vi "DialogRenameVI.vi"(0 "ObjectIn":refnum<class "ClassWriterNative.lvclass">, 1 "ProjectItem":refnum<vi>, 5 "error in (no error)":errorcluster) -> (14 "ObjectOut":refnum<class "ClassWriterNative.lvclass">, 15 "Cancelled":bool, 16 "RenameOption":T1, 19 "error out":errorcluster)   [LabVIEW 2020, in "ClassWriterNative.lvclass"]
uses:
  <resource>/Framework/Providers/Open_GDS/ClassProviders/Provider_LvNativeClass/ClassWriterNative_class/ClassWriterNative.lvclass
  <resource>/Framework/Providers/Open_GDS/ClassProviders/Common/LvIcon_class/GDSLvIcon_ColorControl.ctl
  <resource>/Framework/Providers/Open_GDS/ClassProviders/Provider_BaseClassInterface/ClassWriter_class/RenameViOption.ctl
  <vilib>/Utility/miscctls.llb/LVPoint32TypeDef.ctl
  <resource>/Framework/Providers/Open_GDS/ClassProviders/Common/LvClass_class/GDSLvClass_ClassInfo.ctl
  <vilib>/picture/picture.llb/imagedata.ctl
  <vilib>/Utility/miscctls.llb/LVRowAndColumnUnsignedTypeDef.ctl
  <vilib>/Utility/miscctls.llb/LVRowAndColumnTypeDef.ctl
  <resource>/Framework/Providers/Open_GDS/ClassProviders/Common/LvIcon_class/subvis/GDSLvIcon_TextDataType.ctl
  <resource>/Framework/Providers/Open_GDS/ClassProviders/Common/LvIcon_class/GDSLvIcon_WordCompressionType.ctl
  <resource>/Framework/Providers/Open_GDS/ClassProviders/Common/LvIcon_class/GDSLvIcon_TextAlignment.ctl
  <resource>/Framework/Providers/Open_GDS/ClassProviders/Common/IconEditor/private/GDSIconEditor_IconDialog_Input.vi
  e33266fa-32a9-40b1-9528-20f07e315092.vi
  199ea72b-f535-452c-9e4b-10de01594ef7.vi
  7954b8f4-438f-452e-bba7-858d2d00dd58.vi
  107e4fa8-9309-4a95-9ed7-6f3650e7a3ad.vi
  <resource>/Framework/Providers/Open_GDS/ClassProviders/Provider_LvNativeClass/ClassWriterNative_class/ClassWriterNative.lvclass/ClassWriterNative.ctl
  <resource>/Framework/Providers/Open_GDS/ClassProviders/Common/InterfaceLibrary/InterfaceLibrary.lvlib
  <resource>/Framework/Providers/Open_GDS/ClassProviders/Provider_BaseClassInterface/ClassWriter_class/ClassWriter.lvclass
panel:
  out "VIs to rename":i32(listbox) caption="12 VIs will be renamed(File extension changed)"
  out "LibraryName":string caption="Library Name"
  in  "_ShowContextHelp":bool
  in  "Help":bool
  out "ProductPicture":picture
  out "Ballon":cluster{"Text":string}
  in  "_MethodIcons":bool
  out "_IconPreview":picture caption="Icon Preview"
  in  "_Cancel":bool
  in  "_RenameVI":bool
  in  "_HideHeader":bool=TRUE caption="Force Capital Letters"
  in  "_IconSize":u16(ring) caption="Icon Size" items=["Full", "1 c-term high", "2 c-term high", "3 c-term high"]
  in  "_TextAlignment":u16(ring) caption="Text Alignment" items=["Center", "Left", "Right"]
  in  "_MethodIconName":string caption="Body Text"
  in  "_BodyBk":T2 caption="Body Background"
  in  "_BodyText":T2 caption="Body text"
  in  "_FontCompression":enum16{"Auto", "On", "Off"}(ring) caption="Font Compression"
  in  "_CapitalOnly":bool=TRUE caption="Force Capital Letters"
  out "_After":picture caption="New"
  out "_Before":picture caption="Current"
  out "_VIPath":path caption="VI Path"
  in  "NewName":string caption="New Name"
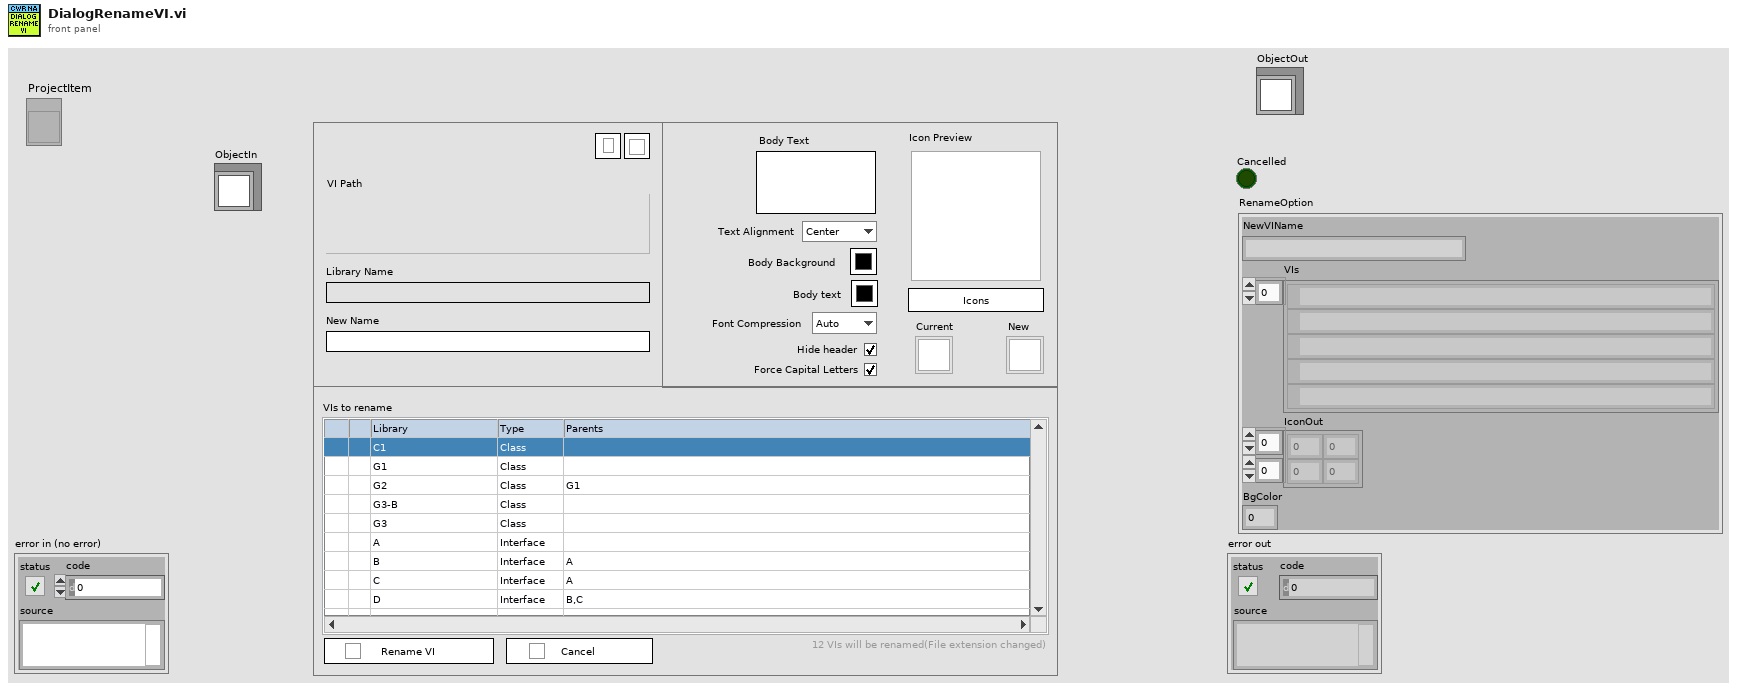
[diagram p1: front panel]
types:
  T1 = typedef "ClassWriter.lvclass/RenameViOption.ctl" = cluster{"NewVIName":string, "VIs":path[], "IconOut":u8[][], "BgColor":u8}
  T2 = typedef "GDSLvIcon_ColorControl.ctl" = cluster{"Decal":bool, "Color":u32}
  T3 = typedef "imagedata.ctl" = cluster{"image type":i32, "image depth":i32, "image":u8[], "mask":u8[], "colors":u32[], "Rectangle":cluster{"left":i16, "top":i16, "right":i16, "bottom":i16}}
  T4 = typedef "LVPoint32TypeDef.ctl" = cluster{"Horizontal":i32, "Vertical":i32}
  T5 = typedef "GDSLvClass_ClassInfo.ctl" = cluster{"Path":path, "Name":string, "QualifiedName":string}
  T6 = cluster{"ClassIndex":i32, "NewName":string, "Cancelled":bool, "VIref":refnum<vi>, "Class":refnum<vi>, "ClassPath":path, "VIPath":path, "Classes":cluster{i32, refnum<vi>, cluster{"Path":path, "Name":string, "QualifiedName":string}[]}[], "ClassInfos":cluster{"ClassName":string, "ViRelPath":path, "AllVIs":string[], "VI-Path":path, "Private":bool}[], "TreeTags":string[], "Selected":i32[], "CurrentIcon":cluster{"BgIcon":u8[][], "BgIconOffset":cluster{"X":i32, "Y":i32}, "BgIconMask":u8[], "ColorsOkayforiconToBeOnTopOf":u8[]}, "StartIconSize":u16, "Offset":cluster{"X":i32, "Y":i32}, "OldOffset":cluster{"X":i32, "Y":i32}, "ConnectorPaneHeight":i32[], "BodyIcon":u8[][], "Icon exist":bool, "HeaderIcon":u8[][], "BodyIconWidth":i32, "BodyIconHeight":i32, "Frame thickness":i32, "StartRow":i32, "FrameColor":u32, "TextBounds":cluster{"FirstRow":i32, "FirstColumn":i32, "LastRow":i32, "LastColumn":i32}, "Header exists":bool, "HeaderBkColor":u32, "DraggingText":bool, "StartTextDraggingPos":T4, "IconSelected":i32, "BgIconOffset":cluster{"X":i32, "Y":i32}, "IconDropped":i32, "Moving":bool, "Folders":path[], "IconPos":cluster{"left":i16, "top":i16, "right":i16, "bottom":i16}[], "IconPaths":cluster{i32, "path out":path}[], "IconNames":string[], "BgIcon":u8[][], "BgIconMask":u8[], "StartTime":i32, "FileExtension":string, "SelectedItems":bool[], "OrgName":string, "ClassVIs":cluster{"Class":refnum<vi>, "ClassInfo":T5, "InheritanceHierarchy":T5[], "ViFullPath":path, "IconPath":path}[], "InterfaceVIs":cluster{"Class":refnum<vi>, "ClassInfo":T5, "InheritanceHierarchy":T5[], "ViFullPath":path, "IconPath":path}[], "Interface":bool, "AllInterfaces":refnum<vi>[], "RowStart(0)":i32, "ImageRows(32)":i32, "AllClasses":refnum<vi>[], "RenameOption":T1}
  T7 = cluster{"Child Text":string[], "Child Tag":string, "Item Indent":i32, "Child Only?":bool, "Glyph Index":i32}[]
  T8 = typedef "LVRowAndColumnTypeDef.ctl" = cluster{"Row":i32, "Column":i32}
  T9 = typedef "LVRowAndColumnUnsignedTypeDef.ctl" = cluster{"Row":u32, "Column":u32}
  T10 = cluster{"Class Refnum Out":refnum<vi>, "ClassInfo":T5, "InheritanceHierarchy":T5[], "ViFullPath":path, "IconPath":path}
  T11 = typedef "GDSLvIcon_TextDataType.ctl" = cluster{"Text":string, "Allow Only Capital Chars":bool, "Compression":T12, "Alignment":T13}
  T12 = typedef "GDSLvIcon_WordCompressionType.ctl" = enum16{"Auto", "On", "Off"}
  T13 = typedef "GDSLvIcon_TextAlignment.ctl" = enum16{"Center", "Left", "Right"}
  T14 = typedef "GDSIconEditor_IconDialog_Input.vi" = cluster{"HeaderIcon":u8[][], "RowStart(0)":i32, "ImageRows(32)":i32, "FrameThickness(1)":u32, "FrameColor":u32, "IconTextDataType":T11, "BodyTextColor":u32, "BodyBackgroundColor":u32, "BodyIconHeight":i32, "BodyIconWidth":i32, "HeaderBackgroundColor":u32, "BodyIcon":u8[][], "Offset":cluster{"X":i32, "Y":i32}, "CurrentIcon":cluster{"BgIcon":u8[][], "BgIconOffset":cluster{"X":i32, "Y":i32}, "BgIconMask":u8[], "ColorsOkayforiconToBeOnTopOf":u8[]}}
  T15 = cluster{"Class":refnum<vi>, "ClassInfo":T5, "InheritanceHierarchy":T5[], "ViFullPath":path, "IconPath":path}[]
  T16 = enum8{"Enabled", "Disabled", "Disabled and Grayed Out"}
  T17 = cluster{"BgIcon":u8[][], "BgIconOffset":cluster{"X":i32, "Y":i32}, "BgIconMask":u8[], "ColorsOkayforiconToBeOnTopOf":u8[]}
  T18 = cluster{"FirstRow":i32, "FirstColumn":i32, "LastRow":i32, "LastColumn":i32}
  T19 = typedef "eventvkey.ctl" = enum16{"ASCII", "Enter", "Return", "Shift", "Ctrl", "Alt", "Cmd", "Opt", "Caps", "NumLock", "Clear", "Break", "Up", "Down", "Left", "Right", "Insert", "Delete", "Home", "End", "PageUp", "PageDown", "Escape", "Help", "Pause", "ScrollLock", "F1", "F2", "F3", "F4", "F5", "F6", "F7", "F8", "F9", "F10", "F11", "F12", "F13", "F14", "F15", "F16", "F17", "F18", "F19", "F20", "F21", "F22", "F23", "F24", "Play", "VolumeUp", "VolumeDown", "Mute", "Two Byte Char"}
  T20 = cluster{"Shift":bool, "Ctrl":bool, "Alt":bool, "Cmd":bool, "Opt":bool}
  T21 = typedef "LVMouseTypeDef.ctl" = cluster{"Mouse Position":cluster{"X":i32, "Y":i32}, "Mouse Modifiers":cluster{"Button Down":bool, "Shift Mod":bool, "Menu Mod":bool, "Option Mod":bool}}
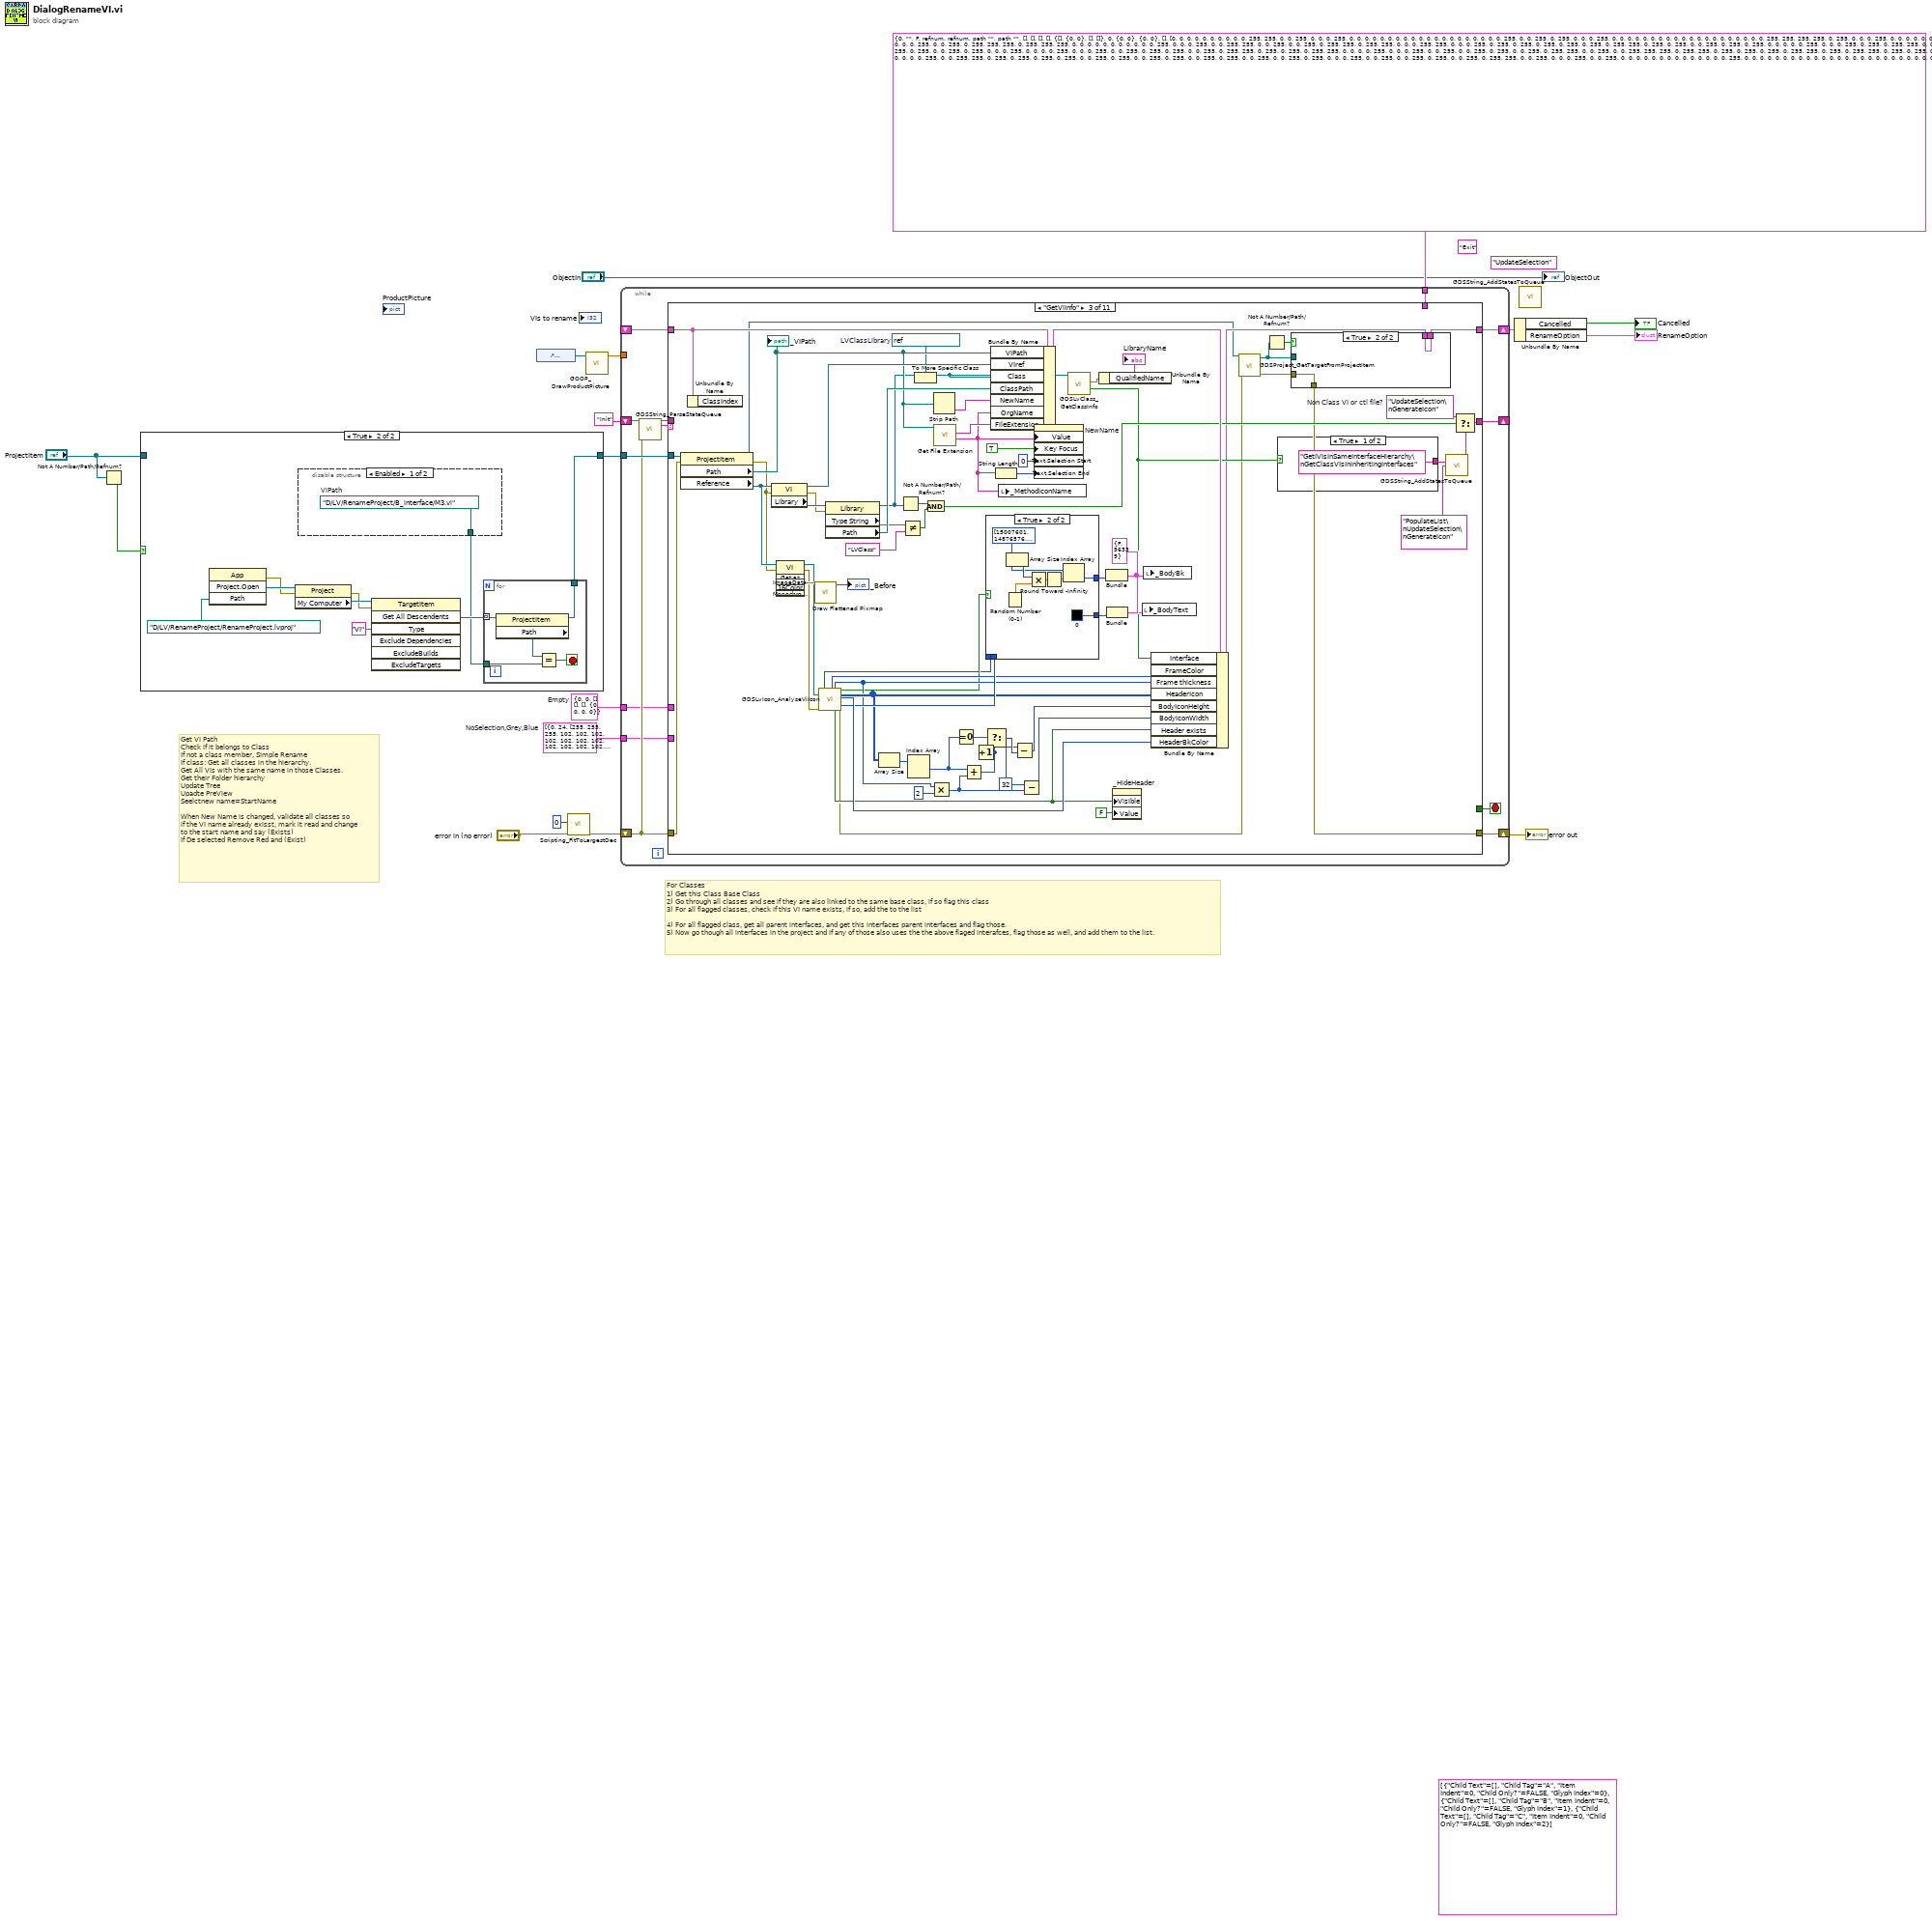
[diagram p0: block diagram]
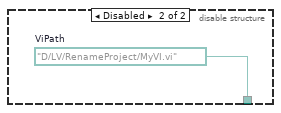
[diagram p3: hidden frame]
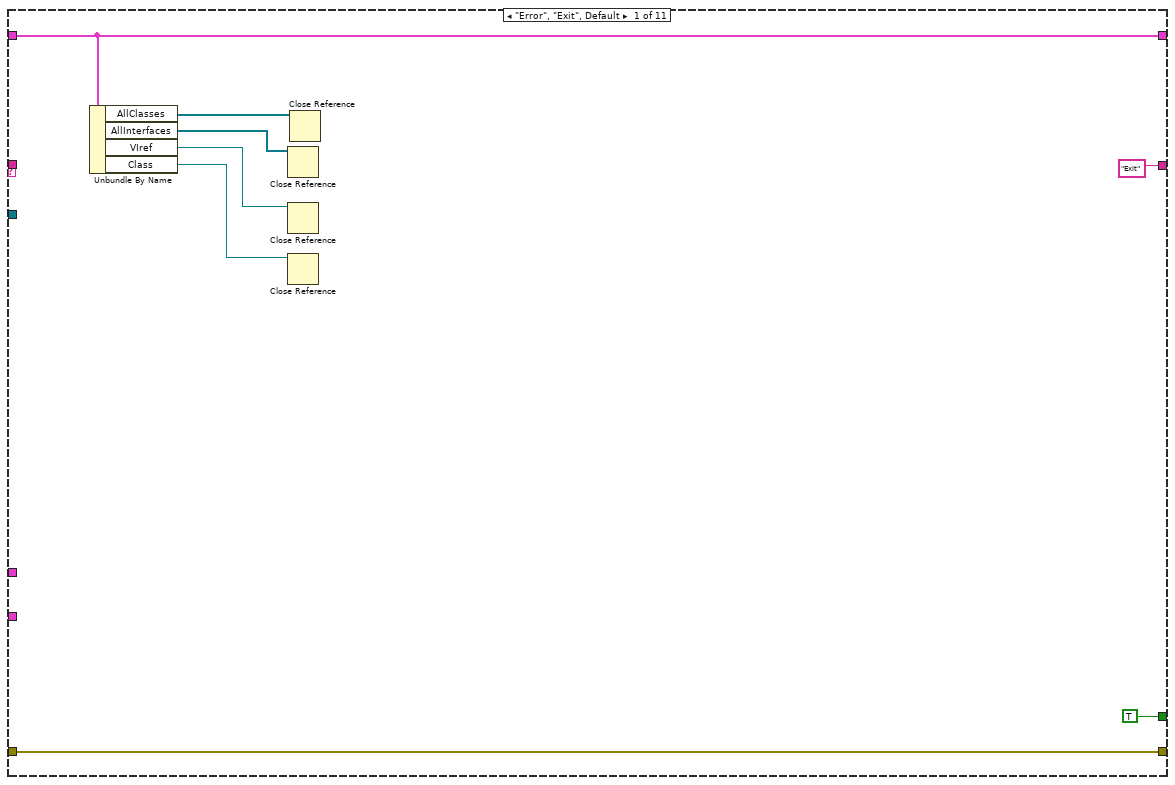
[diagram p4: hidden frame]
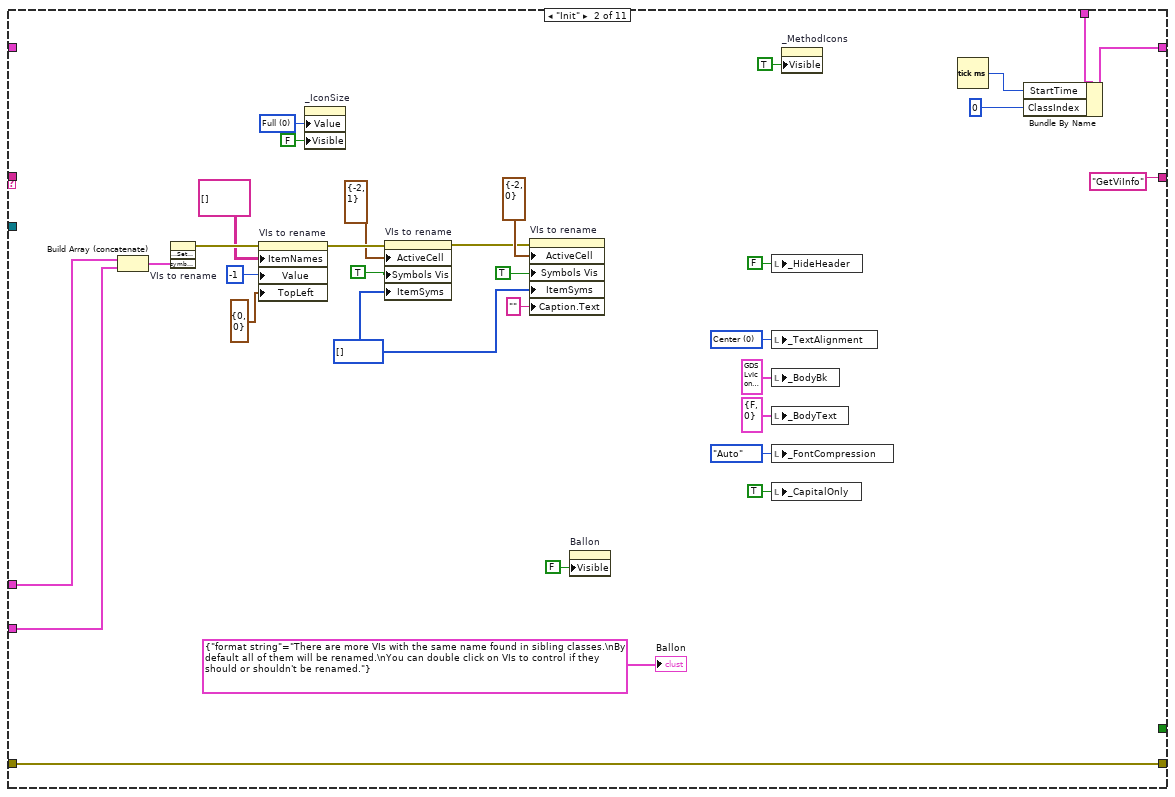
[diagram p5: hidden frame]
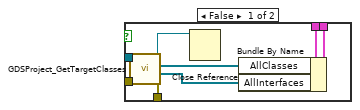
[diagram p6: hidden frame]
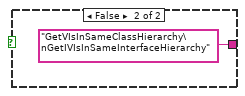
[diagram p7: hidden frame]
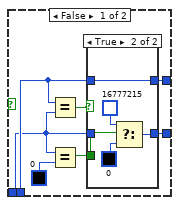
[diagram p8: hidden frame]
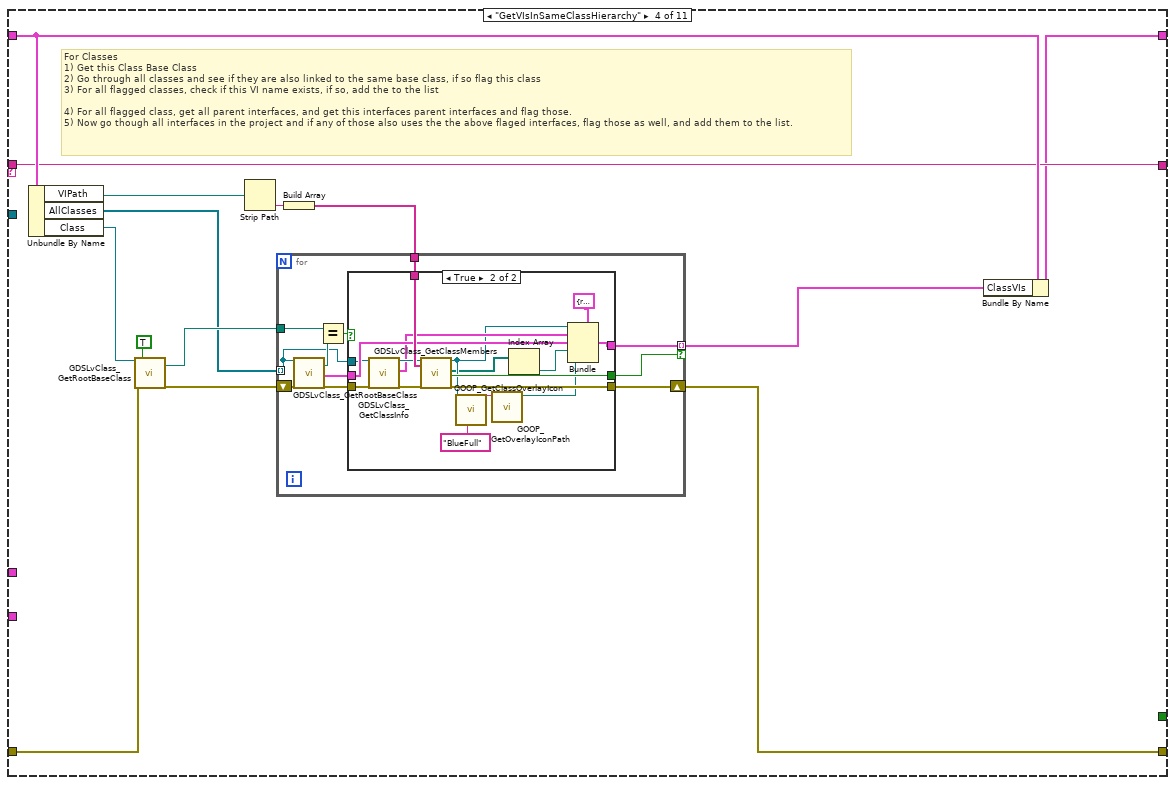
[diagram p10: hidden frame]
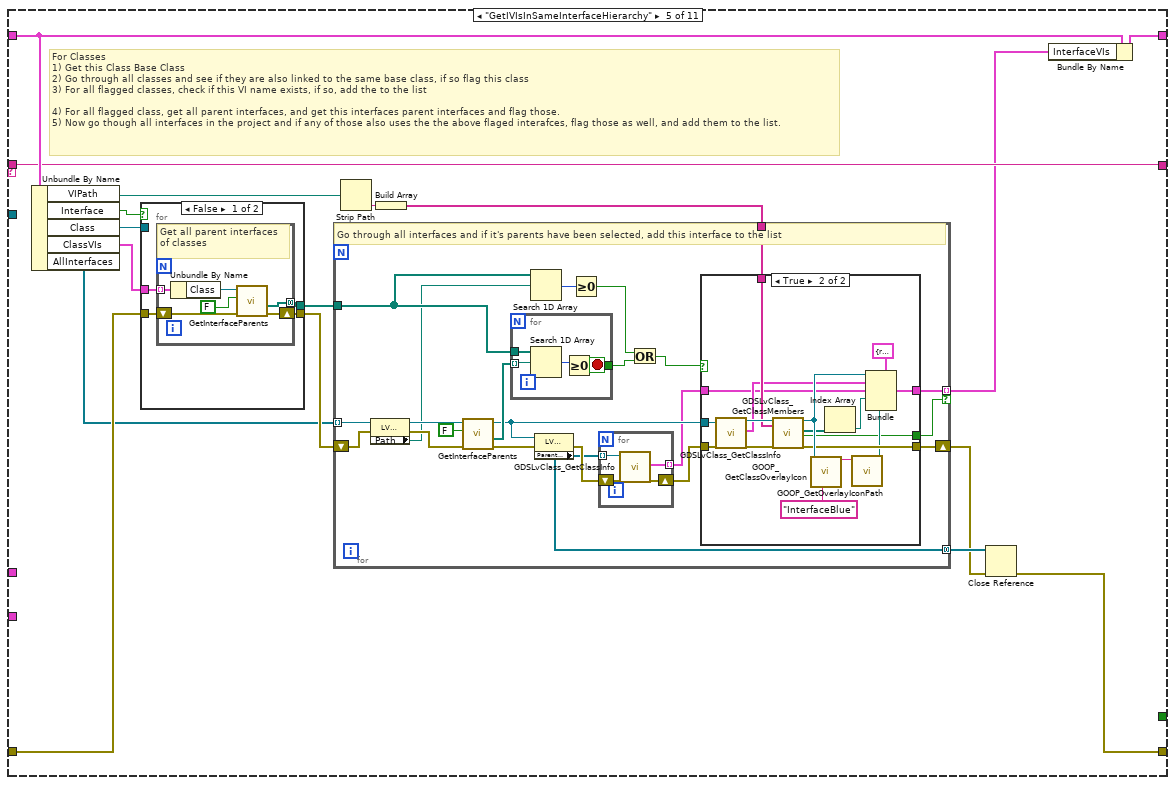
[diagram p12: hidden frame]
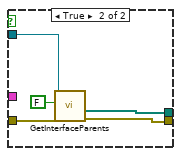
[diagram p13: hidden frame]
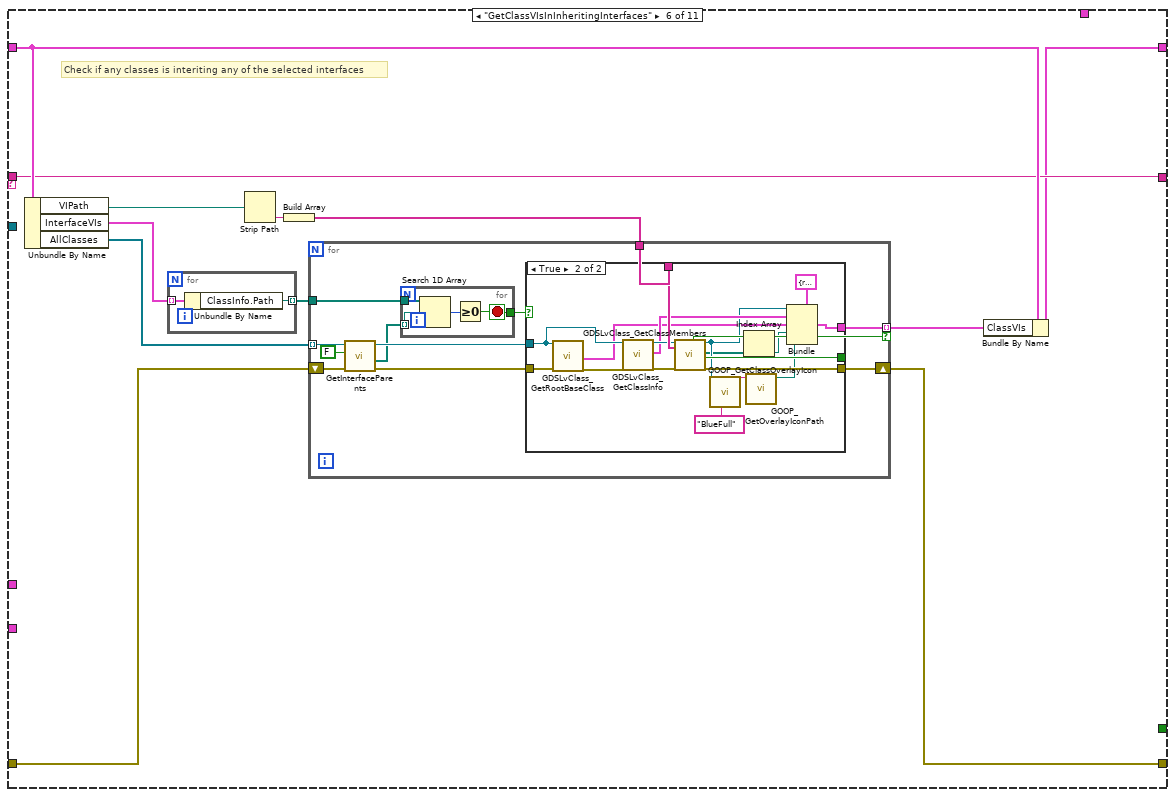
[diagram p15: hidden frame]
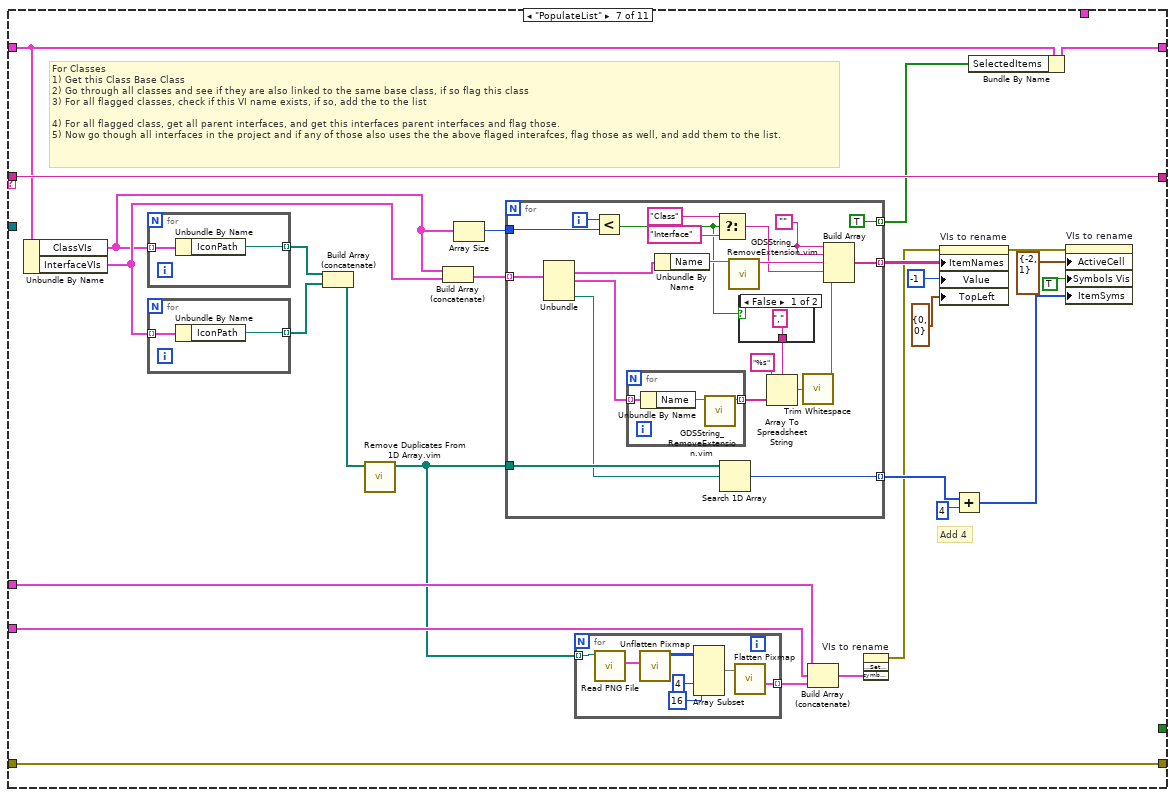
[diagram p17: hidden frame]
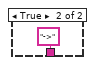
[diagram p18: hidden frame]
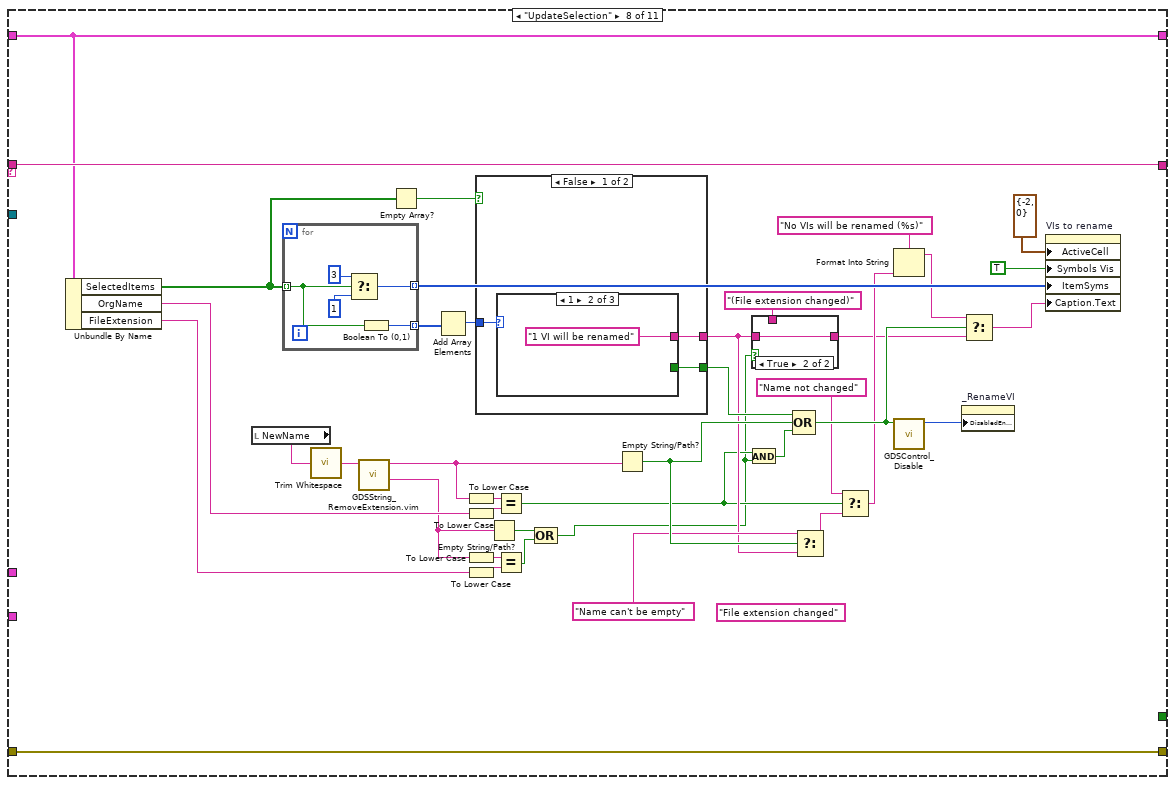
[diagram p19: hidden frame]
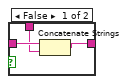
[diagram p20: hidden frame]
diagram:
  w1 = T3 {"image type"=0, "image depth"=0, "image"=[], "mask"=[], "colors"=[], "Rectangle"={"left"=0, "top"=0, "right"=0, "bottom"=0}}  # Empty
  w2 = T3[] [{"image type"=0, "image depth"=24, "image"=[255, 255, 255, 102, 102, 102, 102, 102, 102, 102, 102, 102, 102, 102, 102, 102, 102, 102, 102, 102, 102, 102, 102, 102, 102, 102, 102, 102, 102, 102, 102, 102, 102, 102, 102, 102, 255, 255, 255, 102, 102, 102, 102, 102, 102, 102, 102, 102, 102, 102, 102, 102, 102, 102, 102, 102, 102, 102, 102, 102, 102, 102, 102, 102, 102, 102, 102, 102, 102, 102, 102, 102, 102, 102, 102, 102, 102, 102, 102, 102, 102, 102, 102, 102, 255, 255, 255, 255, 255, 255, 255, 255, 255, 255, 255, 255, 255, 255, 255, 255, 255, 255, 255, 255, 255, 255, 255, 255, 255, 255, 255, 102, 102, 102, 102, 102, 102, 102, 102, 102, 102, 102, 102, 255, 255, 255, 255, 255, 255, 255, 255, 255, 255, 255, 255, 255, 255, 255, 255, 255, 255, 255, 255, 255, 255, 255, 255, 255, 255, 255, 102, 102, 102, 102, 102, 102, 102, 102, 102, 102, 102, 102, 255, 255, 255, 255, 255, 255, 255, 255, 255, 255, 255, 255, 255, 255, 255, 255, 255, 255, 255, 255, 255, 255, 255, 255, 255, 255, 255, 102, 102, 102, 102, 102, 102, 102, 102, 102, 102, 102, 102, 255, 255, 255, 255, 255, 255, 255, 255, 255, 255, 255, 255, 255, 255, 255, 255, 255, 255, 255, 255, 255, 255, 255, 255, 255, 255, 255, 102, 102, 102, 102, 102, 102, 102, 102, 102, 102, 102, 102, 255, 255, 255, 255, 255, 255, 255, 255, 255, 255, 255, 255, 255, 255, 255, 255, 255, 255, 255, 255, 255, 255, 255, 255, 255, 255, 255, 102, 102, 102, 102, 102, 102, 102, 102, 102, 102, 102, 102, 255, 255, 255, 255, 255, 255, 255, 255, 255, 255, 255, 255, 255, 255, 255, 255, 255, 255, 255, 255, 255, 255, 255, 255, 255, 255, 255, 102, 102, 102, 102, 102, 102, 102, 102, 102, 102, 102, 102, 255, 255, 255, 255, 255, 255, 255, 255, 255, 255, 255, 255, 255, 255, 255, 255, 255, 255, 255, 255, 255, 255, 255, 255, 255, 255, 255, 102, 102, 102, 102, 102, 102, 102, 102, 102, 102, 102, 102, 255, 255, 255, 255, 255, 255, 255, 255, 255, 255, 255, 255, 255, 255, 255, 255, 255, 255, 255, 255, 255, 255, 255, 255, 255, 255, 255, 102, 102, 102, 102, 102, 102, 102, 102, 102, 102, 102, 102, 255, 255, 255, 255, 255, 255, 255, 255, 255, 255, 255, 255, 255, 255, 255, 255, 255, 255, 255, 255, 255, 255, 255, 255, 255, 255, 255, 102, 102, 102, 102, 102, 102, 102, 102, 102, 102, 102, 102, 102, 102, 102, 102, 102, 102, 102, 102, 102, 102, 102, 102, 102, 102, 102, 102, 102, 102, 102, 102, 102, 102, 102, 102, 102, 102, 102, 102, 102, 102, 102, 102, 102, 255, 255, 255, 102, 102, 102, 102, 102, 102, 102, 102, 102, 102, 102, 102, 102, 102, 102, 102, 102, 102, 102, 102, 102, 102, 102, 102, 102, 102, 102, 102, 102, 102, 102, 102, 102, 255, 255, 255], "mask"=[255, 248, 255, 248, 255, 248, 255, 248, 255, 248, 255, 248, 255, 248, 255, 248, 255, 248, 255, 248, 255, 248, 255, 248, 255, 248], "colors"=[], "Rectangle"={"left"=0, "top"=0, "right"=13, "bottom"=13}}, {"image type"=0, "image depth"=24, "image"=[255, 255, 255, 143, 143, 143, 143, 143, 143, 143, 143, 143, 143, 143, 143, 143, 143, 143, 143, 143, 143, 143, 143, 143, 143, 143, 143, 143, 143, 143, 143, 143, 143, 143, 143, 143, 255, 255, 255, 143, 143, 143, 143, 143, 143, 143, 143, 143, 143, 143, 143, 143, 143, 143, 143, 143, 143, 143, 143, 143, 143, 143, 143, 143, 143, 143, 143, 143, 143, 143, 143, 143, 170, 170, 170, 143, 143, 143, 143, 143, 143, 143, 143, 143, 143, 143, 143, 143, 143, 143, 143, 143, 143, 143, 143, 143, 143, 143, 143, 143, 143, 143, 143, 143, 143, 143, 143, 143, 170, 170, 170, 211, 211, 211, 143, 143, 143, 143, 143, 143, 143, 143, 143, 143, 143, 143, 143, 143, 143, 143, 143, 143, 143, 143, 143, 143, 143, 143, 143, 143, 143, 143, 143, 143, 170, 170, 170, 232, 232, 232, 255, 255, 255, 143, 143, 143, 143, 143, 143, 143, 143, 143, 143, 143, 143, 143, 143, 143, 143, 143, 143, 143, 143, 143, 143, 143, 143, 143, 143, 143, 170, 170, 170, 232, 232, 232, 255, 255, 255, 211, 211, 211, 143, 143, 143, 143, 143, 143, 143, 143, 143, 158, 158, 158, 143, 143, 143, 143, 143, 143, 143, 143, 143, 143, 143, 143, 170, 170, 170, 232, 232, 232, 255, 255, 255, 211, 211, 211, 143, 143, 143, 143, 143, 143, 143, 143, 143, 211, 211, 211, 218, 218, 218, 158, 158, 158, 143, 143, 143, 143, 143, 143, 170, 170, 170, 232, 232, 232, 255, 255, 255, 211, 211, 211, 154, 154, 154, 143, 143, 143, 143, 143, 143, 143, 143, 143, 226, 226, 226, 255, 255, 255, 218, 218, 218, 158, 158, 158, 170, 170, 170, 232, 232, 232, 255, 255, 255, 211, 211, 211, 154, 154, 154, 143, 143, 143, 143, 143, 143, 143, 143, 143, 143, 143, 143, 165, 165, 165, 226, 226, 226, 255, 255, 255, 218, 218, 218, 232, 232, 232, 255, 255, 255, 211, 211, 211, 154, 154, 154, 143, 143, 143, 143, 143, 143, 143, 143, 143, 143, 143, 143, 143, 143, 143, 143, 143, 143, 165, 165, 165, 226, 226, 226, 255, 255, 255, 255, 255, 255, 211, 211, 211, 154, 154, 154, 143, 143, 143, 143, 143, 143, 143, 143, 143, 143, 143, 143, 143, 143, 143, 143, 143, 143, 143, 143, 143, 143, 143, 143, 165, 165, 165, 226, 226, 226, 211, 211, 211, 154, 154, 154, 143, 143, 143, 143, 143, 143, 143, 143, 143, 143, 143, 143, 143, 143, 143, 143, 143, 143, 143, 143, 143, 143, 143, 143, 143, 143, 143, 143, 143, 143, 165, 165, 165, 154, 154, 154, 143, 143, 143, 143, 143, 143, 143, 143, 143, 143, 143, 143, 143, 143, 143, 143, 143, 143, 143, 143, 143, 255, 255, 255, 143, 143, 143, 143, 143, 143, 143, 143, 143, 143, 143, 143, 143, 143, 143, 143, 143, 143, 143, 143, 143, 143, 143, 143, 143, 143, 143, 143, 143, 143, 143, 143, 143, 255, 255, 255], "mask"=[255, 248, 255, 248, 255, 248, 255, 248, 255, 248, 255, 248, 255, 248, 255, 248, 255, 248, 255, 248, 255, 248, 255, 248, 255, 248], "colors"=[], "Rectangle"={"left"=0, "top"=0, "right"=13, "bottom"=13}}, {"image type"=0, "image depth"=24, "image"=[255, 255, 255, 33, 150, 243, 33, 150, 243, 33, 150, 243, 33, 150, 243, 33, 150, 243, 33, 150, 243, 33, 150, 243, 33, 150, 243, 33, 150, 243, 33, 150, 243, 33, 150, 243, 255, 255, 255, 33, 150, 243, 33, 150, 243, 33, 150, 243, 33, 150, 243, 33, 150, 243, 33, 150, 243, 33, 150, 243, 33, 150, 243, 33, 150, 243, 33, 150, 243, 33, 150, 243, 93, 178, 246, 33, 150, 243, 33, 150, 243, 33, 150, 243, 33, 150, 243, 33, 150, 243, 33, 150, 243, 33, 150, 243, 33, 150, 243, 33, 150, 243, 33, 150, 243, 33, 150, 243, 93, 178, 246, 174, 217, 251, 33, 150, 243, 33, 150, 243, 33, 150, 243, 33, 150, 243, 33, 150, 243, 33, 150, 243, 33, 150, 243, 33, 150, 243, 33, 150, 243, 33, 150, 243, 93, 178, 246, 214, 236, 253, 255, 255, 255, 33, 150, 243, 33, 150, 243, 33, 150, 243, 33, 150, 243, 33, 150, 243, 33, 150, 243, 33, 150, 243, 33, 150, 243, 33, 150, 243, 93, 178, 246, 214, 236, 253, 255, 255, 255, 174, 217, 251, 33, 150, 243, 33, 150, 243, 33, 150, 243, 67, 166, 245, 33, 150, 243, 33, 150, 243, 33, 150, 243, 33, 150, 243, 93, 178, 246, 214, 236, 253, 255, 255, 255, 174, 217, 251, 33, 150, 243, 33, 150, 243, 33, 150, 243, 174, 217, 251, 187, 223, 251, 67, 166, 245, 33, 150, 243, 33, 150, 243, 93, 178, 246, 214, 236, 253, 255, 255, 255, 174, 217, 251, 58, 162, 244, 33, 150, 243, 33, 150, 243, 33, 150, 243, 203, 230, 252, 255, 255, 255, 187, 223, 251, 67, 166, 245, 93, 178, 246, 214, 236, 253, 255, 255, 255, 174, 217, 251, 58, 162, 244, 33, 150, 243, 33, 150, 243, 33, 150, 243, 33, 150, 243, 82, 173, 246, 203, 230, 252, 255, 255, 255, 187, 223, 251, 214, 236, 253, 255, 255, 255, 174, 217, 251, 58, 162, 244, 33, 150, 243, 33, 150, 243, 33, 150, 243, 33, 150, 243, 33, 150, 243, 33, 150, 243, 82, 173, 246, 203, 230, 252, 255, 255, 255, 255, 255, 255, 174, 217, 251, 58, 162, 244, 33, 150, 243, 33, 150, 243, 33, 150, 243, 33, 150, 243, 33, 150, 243, 33, 150, 243, 33, 150, 243, 33, 150, 243, 82, 173, 246, 203, 230, 252, 174, 217, 251, 58, 162, 244, 33, 150, 243, 33, 150, 243, 33, 150, 243, 33, 150, 243, 33, 150, 243, 33, 150, 243, 33, 150, 243, 33, 150, 243, 33, 150, 243, 33, 150, 243, 82, 173, 246, 58, 162, 244, 33, 150, 243, 33, 150, 243, 33, 150, 243, 33, 150, 243, 33, 150, 243, 33, 150, 243, 33, 150, 243, 255, 255, 255, 33, 150, 243, 33, 150, 243, 33, 150, 243, 33, 150, 243, 33, 150, 243, 33, 150, 243, 33, 150, 243, 33, 150, 243, 33, 150, 243, 33, 150, 243, 33, 150, 243, 255, 255, 255], "mask"=[255, 248, 255, 248, 255, 248, 255, 248, 255, 248, 255, 248, 255, 248, 255, 248, 255, 248, 255, 248, 255, 248, 255, 248, 255, 248], "colors"=[], "Rectangle"={"left"=0, "top"=0, "right"=13, "bottom"=13}}]  # NoSelection,Grey,Blue
  (unwired) "UpdateSelection"
  (unwired) "Exit"
  (unwired) T7 [{"Child Text"=[], "Child Tag"="A", "Item Indent"=0, "Child Only?"=FALSE, "Glyph Index"=0}, {"Child Text"=[], "Child Tag"="B", "Item Indent"=0, "Child Only?"=FALSE, "Glyph Index"=1}, {"Child Text"=[], "Child Tag"="C", "Item Indent"=0, "Child Only?"=FALSE, "Glyph Index"=2}] ("Items")
  # "For Classes\n1) Get this Class Base Class\n2) Go through all classes and see if they are also linked to the same base class, if so flag this class\n3) For all flagged classes, check if this VI name exists, if so, add the to the list\n\n4) For all flagged class, get all parent interfaces, and get this interfaces parent interfaces and flag those.\n5) Now go though all interfaces in the project and if any of those also uses the the above flaged interafces, flag those as well, and add them to the list."
  # "Get VI Path\nCheck if it belongs to Class\nIf not a class member, Simple Rename\nIf class: Get all classes in the hierarchy.\nGet All VIs with the same name in those Classes.\nGet their Folder hierarchy\nUpdate Tree\nUpadte PreView\nSeelctnew name=StartName\n\nWhen New Name is changed, validate all classes so\nif the VI name already exisst, mark it read and change\nto the start name and say (Exists)\nIf De selected Remove Red and (Exist)"
  n1 = Not A Number/Path/Refnum?(number/path/refnum="ProjectItem") -> (NaN/Path/Refnum?=w13:bool)
  n2 = case shown="True" w13 {
    tunnel: "ProjectItem" -> [w18 _]
    tunnel: [w18 w22] -> w8
    frame False {
    }
    frame True {
      n3 = invoke class="App" method="Project.Open"("Path"=path "D:/LV/RenameProject/RenameProject.lvproj") -> (error out=w20:errorcluster, "Project:Open"=w26:refnum<vi>)  [unwired: 3 in, 2 out]
      n4 = property class="Project"(reference=w26, error in=w20) -> (error out=w19:errorcluster, "My Computer"=w25:refnum<vi>)  [unwired: 1 out]
      n5 = disable-structure shown="Enabled" {
        disable-tunnel: [w28 w29] -> w21
        frame Enabled {
          w28 = path "D:/LV/RenameProject/B_interface/M3.vi"  # ViPath
        }
        frame Disabled {
          w29 = path "D:/LV/RenameProject/MyVI.vi"  # ViPath
        }
      }
      n6 = invoke class="TargetItem" method="Get All Descendents"(reference=w25, error in=w19, "Type"="VI") -> ("All Descendents"=w23:refnum<vi>[])  [unwired: 4 in, 6 out]
      n7 = for {
        tunnel: w23 -> [w34] mode=indexing
        tunnel: w21 -> [w32]
        tunnel: [w30] -> w22
        stop <- w31 stop-if-true
        n8 = property class="ProjectItem"(reference=w34) -> (reference out=w30:refnum<vi>, "Path"=w33:path)  [unwired: 1 in, 1 out]
        n9 = Equal?(x=w33, y=w32) -> (x = y?=w31:bool)
      }
    }
  }
  n10 = control-ref of="ProductPicture"() -> (w6:refnum<vi>)
  n11 = call <resource>:"Scripting_FitToLargestDec.vi"("error in (no error)"="error in (no error)", "border spacing (2 px)"=0) -> ("error out"=w3:errorcluster)  [unwired: 4 in, 1 out]
  n12 = call <resource>:"GOOP_DrawProductPicture.vi"("ProductPictureControl"=w6) -> ("Zoom Factor"=w7:sgl)  [unwired: 10 in]
  n13 = while {
    shift-right: [w47] -> w15
    shift-left: w3 -> [w39]
    shift-right: [w38] -> _
    shift-left: "Init" -> [w42]
    shift-right: [w43] -> w17
    shift-left: _ -> [w46]
    tunnel: w8 -> [w45]
    tunnel: T6 {"ClassIndex"=0, "NewName"="", "Cancelled"=FALSE, "VIref"=refnum, "Class"=refnum, "ClassPath"=path "", "VIPath"=path "", "Classes"=[], "ClassInfos"=[], "TreeTags"=[], "Selected"=[], "CurrentIcon"={"BgIcon"=[], "BgIconOffset"={"X"=0, "Y"=0}, "BgIconMask"=[], "ColorsOkayforiconToBeOnTopOf"=[]}, "StartIconSize"=0, "Offset"={"X"=0, "Y"=0}, "OldOffset"={"X"=0, "Y"=0}, "ConnectorPaneHeight"=[], "BodyIcon"=[[0, 0, 0, 0, 0, 0, 0, 0, 0, 0, 255, 255, 0, 0, 255, 0, 0, 0, 255, 0, 0, 0, 0, 0, 0, 0, 0, 0, 0, 0], [0, 0, 0, 0, 0, 0, 0, 0, 0, 255, 0, 0, 255, 0, 255, 0, 0, 0, 255, 0, 0, 0, 0, 0, 0, 0, 0, 0, 0, 0], [0, 0, 0, 0, 0, 0, 0, 0, 0, 255, 255, 255, 255, 0, 255, 0, 0, 0, 255, 0, 0, 0, 0, 0, 0, 0, 0, 0, 0, 0], [0, 0, 0, 0, 0, 0, 0, 0, 0, 255, 0, 0, 255, 0, 255, 0, 0, 0, 255, 0, 0, 0, 0, 0, 0, 0, 0, 0, 0, 0], [0, 0, 0, 0, 0, 0, 0, 0, 0, 255, 0, 0, 255, 0, 255, 255, 255, 0, 255, 255, 255, 0, 0, 0, 0, 0, 0, 0, 0, 0], [0, 0, 255, 0, 0, 0, 255, 0, 0, 255, 255, 0, 0, 255, 0, 0, 255, 0, 255, 255, 0, 255, 255, 0, 0, 0, 255, 255, 0, 0], [0, 255, 0, 255, 0, 255, 0, 255, 0, 255, 0, 255, 0, 255, 255, 0, 255, 0, 255, 0, 0, 255, 0, 255, 0, 255, 0, 0, 0, 0], [0, 255, 0, 0, 0, 255, 0, 255, 0, 255, 255, 0, 0, 255, 0, 255, 255, 0, 255, 255, 0, 255, 255, 0, 0, 0, 255, 0, 0, 0], [0, 255, 0, 255, 0, 255, 0, 255, 0, 255, 0, 255, 0, 255, 0, 0, 255, 0, 255, 0, 0, 255, 0, 255, 0, 0, 0, 255, 0, 0], [0, 0, 255, 0, 0, 0, 255, 0, 0, 255, 0, 255, 0, 255, 0, 0, 255, 0, 255, 255, 0, 255, 0, 255, 0, 255, 255, 0, 0, 0], [0, 255, 0, 0, 0, 255, 0, 0, 255, 0, 0, 255, 0, 255, 0, 0, 255, 0, 255, 255, 0, 0, 255, 0, 0, 255, 255, 255, 0, 255], [255, 0, 255, 0, 255, 0, 255, 0, 255, 255, 0, 255, 0, 255, 255, 0, 255, 0, 255, 0, 0, 255, 0, 255, 0, 0, 255, 0, 0, 255], [255, 0, 0, 0, 255, 0, 255, 0, 255, 0, 255, 255, 0, 255, 0, 255, 255, 0, 255, 255, 0, 255, 0, 0, 0, 0, 255, 0, 0, 255], [255, 0, 255, 0, 255, 0, 255, 0, 255, 0, 0, 255, 0, 255, 0, 0, 255, 0, 255, 0, 0, 255, 0, 255, 0, 0, 255, 0, 0, 255], [0, 255, 0, 0, 0, 255, 0, 0, 255, 0, 0, 255, 0, 255, 0, 0, 255, 0, 255, 255, 0, 0, 255, 0, 0, 0, 255, 0, 0, 255], [0, 0, 0, 0, 0, 0, 0, 0, 0, 0, 0, 0, 0, 0, 255, 0, 0, 0, 0, 0, 0, 0, 0, 0, 0, 0, 0, 0, 0, 0], [0, 0, 0, 0, 0, 0, 0, 0, 0, 0, 0, 0, 0, 255, 0, 0, 0, 0, 0, 0, 0, 0, 0, 0, 0, 0, 0, 0, 0, 0], [0, 0, 0, 0, 0, 0, 0, 0, 0, 0, 0, 0, 0, 255, 255, 0, 0, 0, 0, 0, 0, 0, 0, 0, 0, 0, 0, 0, 0, 0], [0, 0, 0, 0, 0, 0, 0, 0, 0, 0, 0, 0, 0, 255, 0, 255, 0, 0, 0, 0, 0, 0, 0, 0, 0, 0, 0, 0, 0, 0], [0, 0, 0, 0, 0, 0, 0, 0, 0, 0, 0, 0, 0, 0, 255, 0, 0, 0, 0, 0, 0, 0, 0, 0, 0, 0, 0, 0, 0, 0], [0, 0, 0, 0, 0, 0, 0, 0, 0, 0, 0, 0, 0, 0, 0, 0, 0, 0, 0, 0, 0, 0, 0, 0, 0, 0, 0, 0, 0, 0], [0, 0, 0, 0, 0, 0, 0, 0, 0, 0, 0, 0, 0, 0, 0, 0, 0, 0, 0, 0, 0, 0, 0, 0, 0, 0, 0, 0, 0, 0]], "Icon exist"=FALSE, "HeaderIcon"=[], "BodyIconWidth"=0, "BodyIconHeight"=0, "Frame thickness"=3, "StartRow"=0, "FrameColor"=0, "TextBounds"={"FirstRow"=2, "FirstColumn"=1, "LastRow"=6, "LastColumn"=27}, "Header exists"=FALSE, "HeaderBkColor"=0, "DraggingText"=FALSE, "StartTextDraggingPos"={"Horizontal"=0, "Vertical"=0}, "IconSelected"=0, "BgIconOffset"={"X"=0, "Y"=0}, "IconDropped"=-1, "Moving"=FALSE, "Folders"=[], "IconPos"=[], "IconPaths"=[], "IconNames"=[], "BgIcon"=[], "BgIconMask"=[], "StartTime"=0, "FileExtension"="", "SelectedItems"=[], "OrgName"="", "ClassVIs"=[], "InterfaceVIs"=[], "Interface"=FALSE, "AllInterfaces"=[], "RowStart(0)"=0, "ImageRows(32)"=32, "AllClasses"=[], "RenameOption"={"NewVIName"="", "VIs"=[], "IconOut"=[], "BgColor"=0}} -> [w44]
    tunnel: w7 -> [_]
    tunnel: w2 -> [w36]
    tunnel: w1 -> [w35]
    stop <- w37 stop-if-true
    n14 = call <resource>:"GDSString_ParseStateQueue.vi"("State Queue"=w42, "Error In (no error)"=w39) -> ("Remaining States"=w40:string, "Current State"=w41:string)  [unwired: 9 in, 3 out]
    n15 = case shown="\"GetViInfo\"" w41 {
      tunnel: w39 -> [w55 w86 w130 w197 w243 w317 w371 w466 w534 w579 w581]
      tunnel: [w55 w86 w92 w191 w234 w314 w371 w466 w499 w563 w580] -> w47
      tunnel: ["Exit" "GetViInfo" w154 w196 w247 w321 w381 w465 w488 w547 w583] -> w38
      tunnel: w46 -> [w52 _ w157 w203 w250 w325 w375 w464 w492 w553 w582]
      tunnel: w45 -> [_ _ w156 _ _ _ _ _ _ _ _]
      tunnel: w44 -> [_ w83 _ _ _ _ _ _ _ _ _]
      tunnel: [w52 w85 w90 w195 w246 w320 w377 w464 w506 w561 w584] -> w43
      tunnel: w40 -> [_ _ _ w196 w247 w321 w381 w465 w488 w547 _]
      tunnel: [TRUE _ _ _ _ _ _ _ _ _ _] -> w37
      tunnel: w36 -> [_ w59 _ _ _ _ w366 _ _ _ _]
      tunnel: w35 -> [_ w60 _ _ _ _ w365 _ _ _ _]
      frame "Error", "Exit", Default {
        n16 = Unbundle By Name(w52) -> ("AllClasses"=w51:refnum<vi>[], "AllInterfaces"=w50:refnum<vi>[], "VIref"=w49:refnum<vi>, "Class"=w48:refnum<vi>)
        n17 = Close Reference(reference=w50) -> ()  [unwired: 1 in, 1 out]
        n18 = Close Reference(reference=w49) -> ()  [unwired: 1 in, 1 out]
        n19 = Close Reference(reference=w48) -> ()  [unwired: 1 in, 1 out]
        n20 = Close Reference(reference=w51) -> ()  [unwired: 1 in, 1 out]
      }
      frame "Init" {
        w57 = i32[] [] ("Item Symbols")
        w79 = u16 0 items=["Center", "Left", "Right"] ("_TextAlignment")
        w81 = u16 0 items=["Full", "1 c-term high", "2 c-term high", "3 c-term high"] ("_IconSize")
        n21 = Build Array (concatenate)(w60, w59) -> (w62:T3[])
        n22 = invoke on="VIs to rename" class="MCListbox (strict)" method="Custom Item Symbols.Set Symbol Array"("symbols"=w62) -> (error out=w61:errorcluster)  [unwired: 3 in, 3 out]
        n23 = property on="VIs to rename" class="MCListbox (strict)"(error in=w61, "ItemNames"=string[][] [] ("Item Names"), "Value"=-1 ("VIs to rename"), "TopLeft"=T9 {"Row"=0, "Column"=0} ("Top Left Visible Cell")) -> (error out=w70:errorcluster)  [unwired: 1 in, 1 out]
        n24 = property on="_IconSize" class="Ring (strict)"("Value"=w81, "Visible"=FALSE) -> ()  [unwired: 2 in, 2 out]
        n25 = property on="VIs to rename" class="MCListbox (strict)"(error in=w70, "ActiveCell"=T8 {"Row"=-2, "Column"=1} ("Active Cell:Active Cell"), "Symbols Vis"=TRUE ("Visible Items:Symbols Visible"), "ItemSyms"=w57) -> (error out=w63:errorcluster)  [unwired: 1 in, 1 out]
        n26 = property on="VIs to rename" class="MCListbox (strict)"(error in=w63, "ActiveCell"=T8 {"Row"=-2, "Column"=0} ("Active Cell:Active Cell"), "Symbols Vis"=TRUE ("Visible Items:Symbols Visible"), "ItemSyms"=w57, "Caption.Text"="") -> ()  [unwired: 1 in, 2 out]
        n27 = property on="Ballon" class="Clust (strict)"("Visible"=FALSE) -> ()  [unwired: 2 in, 2 out]
        n28 = local write "_HideHeader"(FALSE ("_HideHeader")) -> ()
        n29 = local write "_TextAlignment"(w79) -> ()
        n30 = local write "_BodyBk"(T2 {"Decal"=FALSE, "Color"=16774466} ("_BodyBk")) -> ()
        n31 = local write "_BodyText"(T2 {"Decal"=FALSE, "Color"=0} ("_BodyText")) -> ()
        n32 = local write "_FontCompression"(enum16{"Auto", "On", "Off"}."Auto" ("_FontCompression")) -> ()
        n33 = local write "_CapitalOnly"(TRUE ("_CapitalOnly")) -> ()
        n34 = property on="_MethodIcons" class="Bool"("Visible"=TRUE) -> ()  [unwired: 2 in, 2 out]
        n35 = Tick Count (ms)() -> (millisecond timer value=w71:u32)
        n36 = Bundle By Name(cluster=w83, "StartTime"=w71, "ClassIndex"=0 ("Counter")) -> (w85:T6)
        "Ballon" <- cluster{"format string":string} {"format string"="There are more VIs with the same name found in sibling classes.\nBy default all of them will be renamed.\nYou can double click on VIs to control if they should or shouldn't be renamed."} ("Ballon")
      }
      frame "GetViInfo" {
        w106 = refnum<vi> refnum  # LVClassLibrary
        w112 = "UpdateSelection\nGenerateIcon"  # Non Class VI or ctl file?
        w123 = T2 {"Decal"=FALSE, "Color"=56339} ("_BodyBk")
        w132 = u8 32 ("x")
        n37 = property class="ProjectItem"(reference=w156, error in=w130) -> (reference out=w91:refnum<vi>, error out=w114:errorcluster, "Path"=w145:path, "Reference"=w117:refnum<vi>)
        "_VIPath" <- w145
        n38 = Unbundle By Name(w157) -> ()  [unwired: 1 out]
        n39 = property class="VI"(reference=w117, error in=w114) -> (reference out=w151:refnum<vi>, error out=w131:errorcluster, "Library"=w153:refnum<vi>)
        n40 = invoke class="VI" method="VI Icon.Get as Image Data"(reference=w117, error in=w114) -> (reference out=w116:refnum<vi>, error out=w113:errorcluster, "ImageData"=w118:T3)  [unwired: 4 in, 3 out]
        n41 = call <vilib>:"Draw Flattened Pixmap.vi"("image data"=w118) -> ("new picture"=→"_Before":picture)  [unwired: 8 in]
        n42 = call <resource>:"GDSLvIcon_AnalyseViIcon.vi"("ViRef/LvCLassRef/LvLibRef/ViPath/2D_Image"=w116, "error in (no error)"=w113) -> ("BodyTextColor"=w110:u32, "FrameColor"=w125:u32, "FrameThickness(1)"=w126:u32, "ValidHeaderIcon"=w120:bool, "DefaultIcon"=w111:bool, "HeaderIcon"=w127:u8[][], "HeaderBkColor"=w129:u32, "BodyBkColor"=w128:u32, "error out"=w93:errorcluster)  [unwired: 5 in, 4 out]
        n43 = property class="Library"(reference=w153, error in=w131) -> (reference out=w107:refnum<vi>, "Type String"=w108:string, "Path"=w149:path)  [unwired: 1 out]
        n44 = Array Size(array=w127) -> (size(s)=w133:i32[])
        n45 = Not A Number/Path/Refnum?(number/path/refnum=w107) -> (NaN/Path/Refnum?=w155:bool)
        n46 = Not Equal?(x=w108, y="LVClass") -> (x != y?=w150:bool)
        n47 = Index Array(array=w133) -> (element #1=w138:i32)  [unwired: 2 in, 1 out]
        n48 = To More Specific Class(target class=w106, reference=w107) -> (specific class reference=w105:refnum<vi>)  [unwired: 1 in, 1 out]
        n49 = And(x=w155, y=w150) -> (x .and. y?=w101:bool)
        n50 = Multiply(x=w126, y=u8 2) -> (x*y=w137:u32)
        n51 = Strip Path(path=w145) -> (name=w102:string)  [unwired: 1 out]
        n52 = call <vilib>:"Get File Extension.vi"("file"=w145) -> ("filename without extension"=w97:string, "lowercase file extension"=w109:string)  [unwired: 6 in, 3 out]
        n53 = Equal To 0?(x=w138) -> (x = 0?=w139:bool)
        n54 = Add(x=w138, y=w137) -> (x+y=w141:u32)
        n55 = Increment(x=w141) -> (x+1=w140:u32)
        n56 = case shown="True" w111 {
          tunnel: [w174 u32 0] -> w144
          tunnel: [w173 w186] -> w143
          tunnel: w128 -> [w171 _]
          tunnel: w110 -> [w170 _]
          frame False {
            n57 = Equal?(x=w171, y=w170) -> (x = y?=w172:bool)
            n58 = Equal?(x=w170, y=u32 0) -> (x = y?=w175:bool)
            n59 = case shown="True" w172 {
              tunnel: w170 -> [w177 _]
              tunnel: w171 -> [w178 w183]
              tunnel: [w178 w183] -> w173
              tunnel: [w177 w181] -> w174
              tunnel: w175 -> [_ w182]
              frame False {
              }
              frame True {
                n60 = Select(t=u32 16777215, s=w182, f=u32 0) -> (s? t:f=w181:u32)
              }
            }
          }
          frame True {
            w184 = u32[] [15007601, 14876576, 16751729, 15400704, 15507711, 16775072, 12713864, 12124142, 16776704, 16754080, 16752888, 16383904, 7667498, 16754986, 12112639, 3079936, 16776704, 16745561, 9341183, 16746660, 16773906, 2792191, 16762993, 5766954, 16318226, 15517125, 13290186, 10197915, 7442943, 11316396, 9743236, 16757617, 16767648, 6618880, 16711680, 16773906, 65421, 2789375, 13714175, 12827549, 10595204, 7641720, 6062466, 8025242, 11507131, 10386594, 786176, 8584960, 16318208, 16731648, 16755616, 16734715, 14399157, 16754801, 16714752, 10026888, 3524608]
            n61 = Random Number (0-1)() -> (number: 0 to 1=w188:dbl)
            n62 = Array Size(array=w184) -> (size(s)=w185:i32)
            n63 = Multiply(x=w185, y=w188) -> (x*y=w189:dbl)
            n64 = Round Toward -Infinity(1:w189) -> (0:w187:dbl)
            n65 = Index Array(array=w184, index=w187) -> (element=w186:u32)
          }
        }
        n66 = Select(t=w141, s=w139, f=w140) -> (s? t:f=w142:u32)
        n67 = Bundle By Name(cluster=w157, "VIPath"=w145, "VIref"=w151, "Class"=w105, "ClassPath"=w149, "NewName"=w102, "OrgName"=w97, "FileExtension"=w109) -> (w121:T6)
        n68 = String Length(string=w97) -> (length=w146:i32)
        n69 = local write "_MethodIconName"(w97) -> ()
        n70 = Subtract(x=w132, y=w142) -> (x-y=w134:u32)
        n71 = Subtract(x=w132, y=w137) -> (x-y=w135:u32)
        n72 = property on="NewName" class="Str"("Value"=w97, "Key Focus"=TRUE, "Text.Selection Start"=u32 0 ("Text.Selection:Start"), "Text.Selection End"=w146) -> ()  [unwired: 2 in, 2 out]
        n73 = call <resource>:"GDSLvClass_GetClassInfo.vi"("Class Refnum In"=w105) -> ("ClassInfo"=w104:T5, "Is Interface"=w96:bool)  [unwired: 13 in, 4 out]
        n74 = Unbundle By Name(w104) -> ("QualifiedName"=→"LibraryName":string)
        n75 = Bundle(cluster=w123, "Color"=w143) -> (w124:T2)  [unwired: 1 in]
        n76 = Bundle(cluster=w123, "Color"=w144) -> (w122:T2)  [unwired: 1 in]
        n77 = property on="_HideHeader" class="Bool (strict)"("Visible"=w120, "Value"=FALSE ("_HideHeader")) -> ()  [unwired: 2 in, 2 out]
        n78 = local write "_BodyText"(w122) -> ()
        n79 = local write "_BodyBk"(w124) -> ()
        n80 = Bundle By Name(cluster=w121, "Interface"=w96, "FrameColor"=w125, "Frame thickness"=w126, "HeaderIcon"=w127, "BodyIconHeight"=w134, "BodyIconWidth"=w135, "Header exists"=w120, "HeaderBkColor"=w129) -> (w95:T6)
        n81 = call <resource>:"GDSProject_GetTargetFromProjectItem.vi"("error in (no error)"=w93, "ProjectItem in"=w91) -> ("error out"=w94:errorcluster, "TargetItem out"=w89:refnum<vi>)  [unwired: 8 in]
        n82 = Not A Number/Path/Refnum?(number/path/refnum=w89) -> (NaN/Path/Refnum?=w88:bool)
        n83 = case shown="True" w96 {
          tunnel: ["GetIVIsInSameInterfaceHierarchy\nGetClassVIsInInheritingInterfaces" "GetVIsInSameClassHierarchy\nGetIVIsInSameInterfaceHierarchy"] -> w100
          frame True {
          }
          frame False {
          }
        }
        n84 = case shown="True" w88 {
          tunnel: w95 -> [w165 w166]
          tunnel: w94 -> [w164 w167]
          tunnel: [w163 w167] -> w92
          tunnel: [w162 w166] -> w90
          tunnel: w89 -> [w158 _]
          frame False {
            n85 = call <resource>:"GDSProject_GetTargetClasses.vi"("error in (no error)"=w164, "TargetItem in"=w158) -> ("error out"=w163:errorcluster, "LvInterfaces"=w160:refnum<vi>[], "LvClasses"=w161:refnum<vi>[], "TargetItem out"=w159:refnum<vi>)  [unwired: 4 in, 2 out]
            n86 = Close Reference(reference=w159) -> ()  [unwired: 1 in, 1 out]
            n87 = Bundle By Name(cluster=w165, "AllClasses"=w161, "AllInterfaces"=w160) -> (w162:T6)
          }
          frame True {
          }
        }
        n88 = call <resource>:"GDSString_AddStatesToQueue.vi"("State(s) in (\"\")"=w100, "State(s) at Back (\"\")"="PopulateList\nUpdateSelection\nGenerateIcon") -> ("States Out"=w98:string)  [unwired: 13 in]
        n89 = Select(t=w112, s=w101, f=w98) -> (s? t:f=w154:string)
      }
      frame "GetVIsInSameClassHierarchy" {
        # "For Classes\n1) Get this Class Base Class\n2) Go through all classes and see if they are also linked to the same base class, if so flag this class\n3) For all flagged classes, check if this VI name exists, if so, add the to the list\n\n4) For all flagged class, get all parent interfaces, and get this interfaces parent interfaces and flag those.\n5) Now go though all interfaces in the project and if any of those also uses the the above flaged interfaces, flag those as well, and add them to the list."
        n90 = Unbundle By Name(w203) -> ("VIPath"=w201:path, "AllClasses"=w192:refnum<vi>[], "Class"=w202:refnum<vi>)
        n91 = call <resource>:"GDSLvClass_GetRootBaseClass.vi"("ViRef/Path,LvClassRef/Path"=w202, "error in (no error)"=w197, "Don'tOpenReference"=TRUE) -> ("RootBaseClassPath"=w204:path, "error out"=w193:errorcluster)  [unwired: 10 in, 5 out]
        n92 = Strip Path(path=w201) -> (name=w200:string)  [unwired: 1 out]
        n93 = Build Array(w200) -> (w199:string[])
        n94 = for {
          tunnel: w192 -> [w211] mode=indexing
          tunnel: w204 -> [w213]
          shift-right: [w208] -> w191
          shift-left: w193 -> [w215]
          tunnel: w199 -> [w209]
          tunnel: [w207] -> w194 mode=indexing if=w205
          n95 = call <resource>:"GDSLvClass_GetRootBaseClass.vi"("ViRef/Path,LvClassRef/Path"=w211, "error in (no error)"=w215) -> ("RootBaseClassPath"=w214:path, "InheritanceHierarchy"=w206:T5[], "error out"=w212:errorcluster)  [unwired: 11 in, 4 out]
          n96 = Equal?(x=w213, y=w214) -> (x = y?=w210:bool)
          n97 = case shown="True" w210 {
            tunnel: w212 -> [w216 w225]
            tunnel: w211 -> [_ w223]
            tunnel: w209 -> [_ w233]
            tunnel: [w216 w232] -> w208
            tunnel: [_ w231] -> w205
            tunnel: [_ w230] -> w207
            tunnel: w206 -> [_ w227]
            frame False {
            }
            frame True {
              n98 = call <resource>:"GDSLvClass_GetClassInfo.vi"("Class Refnum In"=w223, "error in (no error)"=w225) -> ("Class Refnum Out"=w222:refnum<vi>, "ClassInfo"=w221:T5, "error out"=w224:errorcluster)  [unwired: 12 in, 3 out]
              n99 = call <resource>:"GDSLvClass_GetClassMembers.vi"("Class Refnum In"=w222, "VINames"=w233, "error in (no error)"=w224) -> ("Class Refnum Out"=w220:refnum<vi>, "MethodAbsolutePath"=w217:path[], "Found"=w231:bool, "error out"=w232:errorcluster)  [unwired: 12 in, 1 out]
              n100 = call <resource>:"GOOP_GetClassOverlayIcon.vi"("DefaultIconName(BlueFull or InterfaceBlue)"="BlueFull" ("DefaultIconName(BlueFull)"), "LVClassLibrary in"=w220) -> ("IconName"=w229:string)  [unwired: 7 in, 2 out]
              n101 = call <resource>:"GOOP_GetOverlayIconPath.vi"("IconName(NoPngExtension)"=w229) -> ("IconPath"=w228:path)  [unwired: 10 in]
              n102 = Index Array(array=w217) -> (element=w219:path)  [unwired: 1 in]
              n103 = Bundle(cluster=T10 {"Class Refnum Out"=refnum, "ClassInfo"={"Path"=path "", "Name"="", "QualifiedName"=""}, "InheritanceHierarchy"=[], "ViFullPath"=path "", "IconPath"=path ""}, "Class Refnum Out"=w220, "ClassInfo"=w221, "InheritanceHierarchy"=w227, "ViFullPath"=w219, "IconPath"=w228) -> (w230:T10)
            }
          }
        }
        n104 = Bundle By Name(cluster=w203, "ClassVIs"=w194) -> (w195:T6)
      }
      frame "GetIVIsInSameInterfaceHierarchy" {
        # "For Classes\n1) Get this Class Base Class\n2) Go through all classes and see if they are also linked to the same base class, if so flag this class\n3) For all flagged classes, check if this VI name exists, if so, add the to the list\n\n4) For all flagged class, get all parent interfaces, and get this interfaces parent interfaces and flag those.\n5) Now go though all interfaces in the project and if any of those also uses the the above flaged interafces, flag those as well, and add them to the list."
        n105 = Unbundle By Name(w250) -> ("VIPath"=w249:path, "Interface"=w236:bool, "Class"=w235:refnum<vi>, "ClassVIs"=w245:T15, "AllInterfaces"=w238:refnum<vi>[])
        n106 = case shown="False" w236 {
          tunnel: w245 -> [w254 _]
          tunnel: [w253 w263] -> w244
          tunnel: w243 -> [w252 w265]
          tunnel: [w251 w262] -> w242
          tunnel: w235 -> [_ w264]
          frame False {
            n107 = for {
              tunnel: w254 -> [w260] mode=indexing
              tunnel: [w258] -> w251 mode=concatenating
              shift-right: [w256] -> w253
              shift-left: w252 -> [w255]
              # "Get all parent interfaces of classes"
              n108 = Unbundle By Name(w260) -> ("Class"=w259:refnum<vi>)
              n109 = call <resource>:"GetInterfaceParents.vi"("error in (no error)"=w255, "KeepRefsOpen"=FALSE, "LVClassLibrary in"=w259) -> ("error out"=w256:errorcluster, "InterfaceParents(Path)"=w258:path[])  [unwired: 5 in, 2 out]
            }
          }
          frame True {
            n110 = call <resource>:"GetInterfaceParents.vi"("error in (no error)"=w265, "KeepRefsOpen"=FALSE, "LVClassLibrary in"=w264) -> ("error out"=w263:errorcluster, "InterfaceParents(Path)"=w262:path[])  [unwired: 5 in, 2 out]
          }
        }
        n111 = Strip Path(path=w249) -> (name=w248:string)  [unwired: 1 out]
        n112 = Build Array(w248) -> (w241:string[])
        n113 = for {
          tunnel: w238 -> [w275] mode=indexing
          shift-right: [w285] -> w237
          shift-left: w244 -> [w273]
          tunnel: w242 -> [w271]
          tunnel: w241 -> [w284]
          tunnel: [w278] -> w240 mode=indexing if=w277
          tunnel: [w276] -> w239 mode=concatenating
          # "Go through all interfaces and if it's parents have been selected, add this interface to the list"
          n114 = property class="LVClassLibrary"(reference=w275, error in=w273) -> (reference out=w274:refnum<vi>, error out=w272:errorcluster, "Path"=w270:path)
          n115 = call <resource>:"GetInterfaceParents.vi"("error in (no error)"=w272, "KeepRefsOpen"=FALSE, "LVClassLibrary in"=w274) -> ("error out"=w282:errorcluster, "InterfaceParents(Path)"=w286:path[], "LVClassLibrary Out"=w283:refnum<vi>)  [unwired: 5 in, 1 out]
          n116 = for {
            tunnel: w286 -> [w313] mode=indexing
            tunnel: w271 -> [w312]
            tunnel: [w310] -> w267
            stop <- w310 stop-if-true
            n117 = Search 1D Array(1D array=w312, element=w313) -> (index of element=w311:i32)  [unwired: 1 in]
            n118 = Greater Or Equal To 0?(x=w311) -> (x >= 0?=w310:bool)
          }
          n119 = Search 1D Array(1D array=w271, element=w270) -> (index of element=w269:i32)  [unwired: 1 in]
          n120 = property class="LVClassLibrary"(reference=w283, error in=w282) -> (error out=w281:errorcluster, "Parent Interfaces"=w276:refnum<vi>[])  [unwired: 1 out]
          n121 = Greater Or Equal To 0?(x=w269) -> (x >= 0?=w268:bool)
          n122 = for {
            tunnel: w276 -> [w291] mode=indexing
            shift-right: [w289] -> w280
            shift-left: w281 -> [w290]
            tunnel: [w288] -> w279 mode=indexing
            n123 = call <resource>:"GDSLvClass_GetClassInfo.vi"("Class Refnum In"=w291, "error in (no error)"=w290) -> ("ClassInfo"=w288:T5, "error out"=w289:errorcluster)  [unwired: 12 in, 4 out]
          }
          n124 = Or(x=w268, y=w267) -> (x .or. y?=w266:bool)
          n125 = case shown="True" w266 {
            tunnel: w280 -> [w292 w309]
            tunnel: [w292 w298] -> w285
            tunnel: w284 -> [_ w306]
            tunnel: w283 -> [_ w301]
            tunnel: w279 -> [_ w299]
            tunnel: [_ w296] -> w278
            tunnel: [_ w295] -> w277
            frame False {
            }
            frame True {
              n126 = call <resource>:"GDSLvClass_GetClassInfo.vi"("Class Refnum In"=w301, "error in (no error)"=w309) -> ("Class Refnum Out"=w308:refnum<vi>, "ClassInfo"=w300:T5, "error out"=w307:errorcluster)  [unwired: 12 in, 3 out]
              n127 = call <resource>:"GDSLvClass_GetClassMembers.vi"("Class Refnum In"=w308, "VINames"=w306, "error in (no error)"=w307) -> ("Class Refnum Out"=w302:refnum<vi>, "MethodAbsolutePath"=w293:path[], "Found"=w295:bool, "error out"=w298:errorcluster)  [unwired: 12 in, 1 out]
              n128 = call <resource>:"GOOP_GetClassOverlayIcon.vi"("DefaultIconName(BlueFull or InterfaceBlue)"="InterfaceBlue" ("DefaultIconName(BlueFull)"), "LVClassLibrary in"=w302) -> ("IconName"=w304:string)  [unwired: 7 in, 2 out]
              n129 = Index Array(array=w293) -> (element=w294:path)  [unwired: 1 in]
              n130 = call <resource>:"GOOP_GetOverlayIconPath.vi"("IconName(NoPngExtension)"=w304) -> ("IconPath"=w297:path)  [unwired: 10 in]
              n131 = Bundle(cluster=T10 {"Class Refnum Out"=refnum, "ClassInfo"={"Path"=path "", "Name"="", "QualifiedName"=""}, "InheritanceHierarchy"=[], "ViFullPath"=path "", "IconPath"=path ""}, "Class Refnum Out"=w302, "ClassInfo"=w300, "InheritanceHierarchy"=w299, "ViFullPath"=w294, "IconPath"=w297) -> (w296:T10)
            }
          }
        }
        n132 = Close Reference(reference=w239, error in (no error)=w237) -> (error out=w234:errorcluster)
        n133 = Bundle By Name(cluster=w250, "InterfaceVIs"=w240) -> (w246:T6)
      }
      frame "GetClassVIsInInheritingInterfaces" {
        # "Check if any classes is interiting any of the selected interfaces"
        n134 = Unbundle By Name(w325) -> ("VIPath"=w324:path, "InterfaceVIs"=w316:T15, "AllClasses"=w318:refnum<vi>[])
        n135 = for {
          tunnel: w316 -> [w327] mode=indexing
          tunnel: [w326] -> w315 mode=indexing
          n136 = Unbundle By Name(w327) -> ("ClassInfo.Path"=w326:path)
        }
        n137 = Strip Path(path=w324) -> (name=w323:string)  [unwired: 1 out]
        n138 = Build Array(w323) -> (w322:string[])
        n139 = for {
          tunnel: w318 -> [w333] mode=indexing
          shift-right: [w338] -> w314
          shift-left: w317 -> [w334]
          tunnel: w322 -> [w339]
          tunnel: [w337] -> w319 mode=indexing if=w336
          tunnel: w315 -> [w330]
          n140 = call <resource>:"GetInterfaceParents.vi"("error in (no error)"=w334, "KeepRefsOpen"=FALSE, "LVClassLibrary in"=w333) -> ("error out"=w332:errorcluster, "InterfaceParents(Path)"=w329:path[], "LVClassLibrary Out"=w331:refnum<vi>)  [unwired: 5 in, 1 out]
          n141 = for {
            tunnel: w330 -> [w343]
            tunnel: w329 -> [w342] mode=indexing
            tunnel: [w340] -> w328
            stop <- w340 stop-if-true
            n142 = Search 1D Array(1D array=w343, element=w342) -> (index of element=w341:i32)  [unwired: 1 in]
            n143 = Greater Or Equal To 0?(x=w341) -> (x >= 0?=w340:bool)
          }
          n144 = case shown="True" w328 {
            tunnel: w332 -> [w344 w351]
            tunnel: w331 -> [_ w350]
            tunnel: w339 -> [_ w362]
            tunnel: [w344 w361] -> w338
            tunnel: [_ w360] -> w336
            tunnel: [_ w359] -> w337
            frame False {
            }
            frame True {
              n145 = call <resource>:"GDSLvClass_GetRootBaseClass.vi"("ViRef/Path,LvClassRef/Path"=w350, "error in (no error)"=w351) -> ("InheritanceHierarchy"=w348:T5[], "error out"=w349:errorcluster)  [unwired: 11 in, 5 out]
              n146 = call <resource>:"GDSLvClass_GetClassInfo.vi"("Class Refnum In"=w350, "error in (no error)"=w349) -> ("Class Refnum Out"=w354:refnum<vi>, "ClassInfo"=w353:T5, "error out"=w355:errorcluster)  [unwired: 12 in, 3 out]
              n147 = call <resource>:"GDSLvClass_GetClassMembers.vi"("Class Refnum In"=w354, "VINames"=w362, "error in (no error)"=w355) -> ("Class Refnum Out"=w352:refnum<vi>, "MethodAbsolutePath"=w345:path[], "Found"=w360:bool, "error out"=w361:errorcluster)  [unwired: 12 in, 1 out]
              n148 = call <resource>:"GOOP_GetClassOverlayIcon.vi"("DefaultIconName(BlueFull or InterfaceBlue)"="BlueFull" ("DefaultIconName(BlueFull)"), "LVClassLibrary in"=w352) -> ("IconName"=w358:string)  [unwired: 7 in, 2 out]
              n149 = Index Array(array=w345) -> (element=w347:path)  [unwired: 1 in]
              n150 = call <resource>:"GOOP_GetOverlayIconPath.vi"("IconName(NoPngExtension)"=w358) -> ("IconPath"=w357:path)  [unwired: 10 in]
              n151 = Bundle(cluster=T10 {"Class Refnum Out"=refnum, "ClassInfo"={"Path"=path "", "Name"="", "QualifiedName"=""}, "InheritanceHierarchy"=[], "ViFullPath"=path "", "IconPath"=path ""}, "Class Refnum Out"=w352, "ClassInfo"=w353, "InheritanceHierarchy"=w348, "ViFullPath"=w347, "IconPath"=w357) -> (w359:T10)
            }
          }
        }
        n152 = Bundle By Name(cluster=w325, "ClassVIs"=w319) -> (w320:T6)
      }
      frame "PopulateList" {
        # "Add 4"
        # "For Classes\n1) Get this Class Base Class\n2) Go through all classes and see if they are also linked to the same base class, if so flag this class\n3) For all flagged classes, check if this VI name exists, if so, add the to the list\n\n4) For all flagged class, get all parent interfaces, and get this interfaces parent interfaces and flag those.\n5) Now go though all interfaces in the project and if any of those also uses the the above flaged interafces, flag those as well, and add them to the list."
        n153 = Unbundle By Name(w375) -> ("ClassVIs"=w369:T15, "InterfaceVIs"=w370:T15)
        n154 = for {
          tunnel: w369 -> [w427] mode=indexing
          tunnel: [w426] -> w374 mode=indexing
          n155 = Unbundle By Name(w427) -> ("IconPath"=w426:path)
        }
        n156 = for {
          tunnel: w370 -> [w391] mode=indexing
          tunnel: [w390] -> w373 mode=indexing
          n157 = Unbundle By Name(w391) -> ("IconPath"=w390:path)
        }
        n158 = Build Array (concatenate)(w374, w373) -> (w372:path[])
        n159 = call "Remove Duplicates From 1D Array.vim"("array"=w372) -> ("array with duplicates removed"=w364:path[])  [unwired: 10 in]
        n160 = Build Array (concatenate)(w369, w370) -> (w367:T15)
        n161 = Array Size(array=w369) -> (size(s)=w368:i32)
        n162 = for {
          tunnel: w367 -> [w420] mode=indexing
          tunnel: [w412] -> w386 mode=indexing
          tunnel: w364 -> [w411]
          tunnel: [w410] -> w379 mode=indexing
          tunnel: [TRUE] -> w376 mode=indexing
          tunnel: w368 -> [w405]
          i -> [w406]
          w418 = ""
          n163 = Unbundle(w420) -> ("ClassInfo"=w400:T5, "InheritanceHierarchy"=w401:T5[], "IconPath"=w399:path)  [unwired: 2 out]
          n164 = Less?(x=w406, y=w405) -> (x < y?=w402:bool)
          n165 = for {
            tunnel: w401 -> [w425] mode=indexing
            tunnel: [w423] -> w416 mode=indexing
            n166 = Unbundle By Name(w425) -> ("Name"=w424:string)
            n167 = call "GDSString_RemoveExtension.vim"("NameWithExtension"=w424) -> ("NameWithoutExtension"=w423:string)  [unwired: 9 in, 1 out]
          }
          n168 = Unbundle By Name(w400) -> ("Name"=w419:string)
          n169 = Select(t="Class", s=w402, f="Interface") -> (s? t:f=w404:string)
          n170 = Search 1D Array(1D array=w411, element=w399) -> (index of element=w410:i32)  [unwired: 1 in]
          n171 = call "GDSString_RemoveExtension.vim"("NameWithExtension"=w419) -> ("NameWithoutExtension"=w417:string)  [unwired: 9 in, 1 out]
          n172 = case shown="False" w402 {
            tunnel: ["," ("delimiter (Tab)") "->" ("delimiter (Tab)")] -> w414
            frame False {
            }
            frame True {
            }
          }
          n173 = Array To Spreadsheet String(delimiter (Tab)=w414, array=w416, 3:"%s" ("format string")) -> (spreadsheet string=w413:string)
          n174 = call <vilib>:"Trim Whitespace.vi"("string"=w413) -> ("trimmed string"=w403:string)  [unwired: 1 in]
          n175 = Build Array(w418, w418, w417, w404, w403) -> (w412:string[])
        }
        n176 = for {
          tunnel: w364 -> [w398] mode=indexing
          tunnel: [w392] -> w389 mode=indexing
          n177 = call <vilib>:"Read PNG File.vi"("path to PNG file"=w398) -> ("image data"=w397:T3)  [unwired: 8 in, 2 out]
          n178 = call <vilib>:"Unflatten Pixmap.vi"("image data"=w397) -> ("24-bit pixmap"=w396:u32[][])  [unwired: 4 in, 6 out]
          n179 = Array Subset(array=w396, index (col)=4 ("index"), length (col)=16 ("length")) -> (w393:u32[][])  [unwired: 2 in]
          n180 = call <vilib>:"Flatten Pixmap.vi"("24-bit pixmap"=w393) -> ("image data"=w392:T3)  [unwired: 10 in]
        }
        n181 = Build Array (concatenate)(w365, w366, w389) -> (w388:T3[])
        n182 = invoke on="VIs to rename" class="MCListbox (strict)" method="Custom Item Symbols.Set Symbol Array"("symbols"=w388) -> (error out=w363:errorcluster)  [unwired: 3 in, 3 out]
        n183 = property on="VIs to rename" class="MCListbox (strict)"(error in=w363, "ItemNames"=w386, "Value"=-1 ("VIs to rename"), "TopLeft"=T9 {"Row"=0, "Column"=0} ("Top Left Visible Cell")) -> (error out=w382:errorcluster)  [unwired: 1 in, 1 out]
        n184 = Add(x=w379, y=4 ("index")) -> (x+y=w378:i32[])
        n185 = Bundle By Name(cluster=w375, "SelectedItems"=w376) -> (w377:T6)
        n186 = property on="VIs to rename" class="MCListbox (strict)"(error in=w382, "ActiveCell"=T8 {"Row"=-2, "Column"=1} ("Active Cell:Active Cell"), "Symbols Vis"=TRUE ("Visible Items:Symbols Visible"), "ItemSyms"=w378) -> ()  [unwired: 1 in, 2 out]
      }
      frame "UpdateSelection" {
        (unwired) "File extension changed"
        n187 = Unbundle By Name(w464) -> ("SelectedItems"=w442:bool[], "OrgName"=w451:string, "FileExtension"=w438:string)
        n188 = local read "NewName"() -> (w457:string)
        n189 = for {
          tunnel: w442 -> [w482] mode=indexing
          tunnel: [w483] -> w461 mode=indexing
          tunnel: [w481] -> w460 mode=indexing
          n190 = Select(t=3 ("index"), s=w482, f=1 ("index")) -> (s? t:f=w483:i32)
          n191 = Boolean To (0,1)(Boolean=w482) -> (0, 1=w481:i16)
        }
        n192 = call <vilib>:"Trim Whitespace.vi"("string"=w457) -> ("trimmed string"=w455:string)  [unwired: 1 in]
        n193 = call "GDSString_RemoveExtension.vim"("NameWithExtension"=w455) -> ("Extension"=w431:string, "NameWithoutExtension"=w454:string)  [unwired: 9 in]
        n194 = Empty Array?(array=w442) -> (empty?=w441:bool)
        n195 = Add Array Elements(numeric array=w460) -> (sum=w459:i16)
        n196 = To Lower Case(string=w454) -> (all lower case string=w453:string)
        n197 = To Lower Case(string=w451) -> (all lower case string=w452:string)
        n198 = To Lower Case(string=w431) -> (all lower case string=w439:string)
        n199 = To Lower Case(string=w438) -> (all lower case string=w440:string)
        n200 = case shown="False" w441 {
          tunnel: w459 -> [w473 _]
          tunnel: [w472 _] -> w456
          tunnel: [w471 "This VI will be renamed"] -> w436
          frame False {
            n201 = case shown="1" w473 {
              selector: w473 -> [_ _ w479]
              tunnel: [TRUE _ _] -> w472
              tunnel: ["No VIs selected" "1 VI will be renamed" w477] -> w471
              frame 0, Default {
              }
              frame 1 {
              }
              frame 2.. {
                n202 = Format Into String(format string="%d VIs will be renamed", w479) -> (resulting string=w477:string)  [unwired: 2 in, 1 out]
              }
            }
          }
          frame True {
          }
        }
        n203 = Empty String/Path?(string/path=w431) -> (empty?=w430:bool)
        n204 = Equal?(x=w453, y=w452) -> (x = y?=w433:bool)
        n205 = Equal?(x=w439, y=w440) -> (x = y?=w429:bool)
        n206 = Compound Arithmetic op=OR(w430, w429) -> (w428:bool)
        n207 = Empty String/Path?(string/path=w454) -> (empty?=w446:bool)
        n208 = And(x=w433, y=w428) -> (x .and. y?=w432:bool)
        n209 = case shown="True" w428 {
          tunnel: w436 -> [w469 w470]
          tunnel: [w468 w470] -> w435
          tunnel: "(File extension changed)" -> [w467 _]
          frame False {
            n210 = Concatenate Strings(w469, w467) -> (w468:string)
          }
          frame True {
          }
        }
        n211 = Compound Arithmetic op=OR(w456, w446, w432) -> (w450:bool)
        n212 = Select(t="Name can't be empty", s=w446, f=w436) -> (s? t:f=w445:string)
        n213 = Select(t="Name not changed", s=w433, f=w445) -> (s? t:f=w443:string)
        n214 = Format Into String(format string="No VIs will be renamed (%s)", w443) -> (resulting string=w447:string)  [unwired: 2 in, 1 out]
        n215 = call <resource>:"GDSControl_Disable.vi"("Disasble(True)"=w450) -> ("Enable Property"=w458:T16)  [unwired: 10 in]
        n216 = property on="_RenameVI" class="Bool"("DisabledEnum"=w458) -> ()  [unwired: 2 in, 2 out]
        n217 = Select(t=w447, s=w450, f=w435) -> (s? t:f=w449:string)
        n218 = property on="VIs to rename" class="MCListbox (strict)"("ActiveCell"=T8 {"Row"=-2, "Column"=0} ("Active Cell:Active Cell"), "Symbols Vis"=TRUE ("Visible Items:Symbols Visible"), "ItemSyms"=w461, "Caption.Text"=w449) -> ()  [unwired: 2 in, 2 out]
      }
      frame "GenerateIcon" {
        n219 = Unbundle By Name(w492) -> ("CurrentIcon"=w532:T17)
        n220 = Unbundle By Name(w492) -> ("ConnectorPaneHeight"=w528:i32[], "BodyIconHeight"=w529:i32, "BodyIconWidth"=w531:i32)
        n221 = Unbundle By Name(w492) -> ("StartIconSize"=w511:u16, "StartRow"=w514:i32, "FrameColor"=w507:u32, "Frame thickness"=w508:i32, "HeaderIcon"=w509:u8[][])
        n222 = local read "_IconSize"() -> (w498:u16)
        n223 = local read "_HideHeader"() -> (w530:bool)
        n224 = local read "_BodyBk"() -> (w496:T2)
        n225 = Unbundle By Name(w492) -> ("HeaderBkColor"=w491:u32)
        n226 = Unbundle By Name(w496) -> ("Color"=w493:u32)
        n227 = call <resource>:"GDSIconEditor_IconSizeAdjustment.vi"("BodyIconHeightIn"=w529, "HideHeader"=w530, "ConnectorPaneHeight"=w528, "Frame thickness"=w508, "_IconSize"=w498, "HeaderIconIn"=w509) -> ("HeaderIconOut"=w527:u8[][], "BodyIconHeightOut"=w526:u32, "ImageRows"=w489:i32)  [unwired: 3 in]
        n228 = Not Equal?(x=w511, y=w498) -> (x != y?=w512:bool)
        n229 = call <resource>:"GDSLvIcon_Convert24bitTo8bitColor.vi"("Color 24bit In"=w491) -> ("Color out(256)"=w497:u8)  [unwired: 15 in, 3 out]
        n230 = call <resource>:"GDSLvIcon_Convert24bitTo8bitColor.vi"("Color 24bit In"=w493) -> ("Color out(256)"=w486:u8)  [unwired: 15 in, 3 out]
        n231 = Select(t=0, s=w512, f=w514) -> (s? t:f=w490:i32)
        n232 = local read "_FontCompression"() -> (w537:enum16{"Auto", "On", "Off"})
        n233 = local read "_MethodIconName"() -> (w521:string)
        n234 = local read "_CapitalOnly"() -> (w536:bool)
        n235 = local read "_TextAlignment"() -> (w535:u16)
        n236 = Build Array(w497, w486) -> (w494:u8[])
        n237 = local read "_BodyText"() -> (w533:T2)
        n238 = Unbundle By Name(w492) -> ("OldOffset.X"=w516:i32, "OldOffset.Y"=w519:i32)  [unwired: 1 out]
        n239 = Unbundle By Name(w492) -> ("Offset"=w500:cluster{"X":i32, "Y":i32})
        n240 = Bundle By Name(cluster=w532, "ColorsOkayforiconToBeOnTopOf"=w494) -> (w495:T17)
        n241 = Bundle By Name(cluster=T11 {"Text"="", "Allow Only Capital Chars"=FALSE, "Compression"=enum."Auto", "Alignment"=enum."Center"} ("Text"), "Alignment"=w535, "Text"=w521, "Allow Only Capital Chars"=w536, "Compression"=w537) -> (w522:T11)
        n242 = Unbundle(w533) -> ("Color"=w542:u32)  [unwired: 1 out]
        n243 = Unbundle By Name(w500) -> ("X"=w517:i32, "Y"=w520:i32)
        n244 = call <resource>:"GDSLvIcon_GenerateIconText.vi"("Text"=w522, "TextPixelHeight(5-30)"=w526, "Foreground color"=w542, "Background color"=w493, "error in (no error)"=w534, "Offset"=w500, "Text Pixel width(32-FrameThicknes*2))"=w531) -> ("X-Limited"=w505:bool, "Y-Limited"=w504:bool, "TextOut"=w501:u8[][], "TextBounds"=w523:T18, "error out"=w544:errorcluster)  [unwired: 8 in]
        n245 = Select(t=w516, s=w505, f=w517) -> (s? t:f=w515:i32)
        n246 = Select(t=w519, s=w504, f=w520) -> (s? t:f=w518:i32)
        n247 = call <resource>:"GDSLvIcon_CreateIconPicture.vi"("FrameColor"=w507, "FrameThickness(1)"=w508, "HeaderIconIn"=w527, "BodyIconIn"=w501, "error in (no error)"=w544, "ImageRows(32)"=w489, "BigSizeIcon(x6)"=4, "RowStart(0)"=w490, "BgIcon"=w495) -> ("BodyIconOut"=w487:u8[][], "IconPictureOut"=→"_After":picture, "LargeIconPictureOut(x6)"=→"_IconPreview":picture, "BodyOffset"=w538:cluster{"X":i32, "Y":i32}, "error out"=w499:errorcluster)  [unwired: 5 in, 1 out]
        n248 = Unbundle(w538) -> ("X"=w539:i32, "Y"=w540:i32)
        n249 = Bundle("Y"=w540, "X"=w539, "Y"=w540, "X"=w539) -> (w541:cluster{"Y":i32, "X":i32, "Y":i32, "X":i32})  [unwired: 1 in]
        n250 = Add(x=w541, y=w523) -> (x+y=w502:cluster{i32, i32, i32, i32})
        n251 = Bundle By Name(cluster=w492, "Offset.X"=w515, "Offset.Y"=w518, "Icon exist"=TRUE, "BodyIcon"=w501, "RowStart(0)"=w490, "ImageRows(32)"=w489, "TextBounds"=w502, "RenameOption.IconOut"=w487, "RenameOption.BgColor"=w486) -> (w506:T6)
      }
      frame "UpdateIcon" {
        w562 = T17 {"BgIcon"=[], "BgIconOffset"={"X"=0, "Y"=0}, "BgIconMask"=[], "ColorsOkayforiconToBeOnTopOf"=[]}  # BgIcon
        n252 = Unbundle By Name(w553) -> ("StartIconSize"=w567:u16, "StartRow"=w570:i32, "FrameColor"=w566:u32, "Frame thickness"=w552:i32, "HeaderIcon"=w555:u8[][])
        n253 = local read "_IconSize"() -> (w550:u16)
        n254 = Unbundle By Name(w553) -> ("BodyIcon"=w571:u8[][])
        n255 = local read "_BodyBk"() -> (w564:T2)
        n256 = Unbundle By Name(w564) -> ("Color"=w551:u32)
        n257 = Unbundle By Name(w553) -> ("BgIcon"=w572:u8[][], "BgIconOffset"=w573:cluster{"X":i32, "Y":i32}, "BgIconMask"=w575:u8[], "HeaderBkColor"=w576:u32)
        n258 = Not Equal?(x=w567, y=w550) -> (x != y?=w568:bool)
        n259 = call <resource>:"GDSLvIcon_Convert24bitTo8bitColor.vi"("Color 24bit In"=w576) -> ("Color out(256)"=w577:u8)  [unwired: 15 in, 3 out]
        n260 = call <resource>:"GDSLvIcon_Convert24bitTo8bitColor.vi"("Color 24bit In"=w551) -> ("Color out(256)"=w546:u8)  [unwired: 15 in, 3 out]
        n261 = Select(t=0, s=w568, f=w570) -> (s? t:f=w549:i32)
        n262 = Build Array(w577, w546) -> (w574:u8[])
        n263 = Unbundle By Name(w553) -> ("ConnectorPaneHeight"=w556:i32[], "BodyIconHeight"=w557:i32)  [unwired: 1 out]
        n264 = Bundle By Name(cluster=w562, "BgIcon"=w572, "BgIconOffset"=w573, "BgIconMask"=w575, "ColorsOkayforiconToBeOnTopOf"=w574) -> (w578:T17)
        n265 = local read "_HideHeader"() -> (w558:bool)
        n266 = call <resource>:"GDSIconEditor_IconSizeAdjustment.vi"("BodyIconHeightIn"=w557, "HideHeader"=w558, "ConnectorPaneHeight"=w556, "Frame thickness"=w552, "_IconSize"=w550, "HeaderIconIn"=w555) -> ("HeaderIconOut"=w554:u8[][], "ImageRows"=w548:i32)  [unwired: 3 in, 1 out]
        n267 = call <resource>:"GDSLvIcon_CreateIconPicture.vi"("FrameColor"=w566, "FrameThickness(1)"=w552, "HeaderIconIn"=w554, "BodyIconIn"=w571, "error in (no error)"=w579, "ImageRows(32)"=w548, "BigSizeIcon(x6)"=4, "RowStart(0)"=w549, "BgIcon"=w578) -> ("BodyIconOut"=w545:u8[][], "IconPictureOut"=w560:picture, "LargeIconPictureOut(x6)"=w559:picture, "error out"=w563:errorcluster)  [unwired: 5 in, 2 out]
        n268 = Bundle By Name(cluster=w553, "CurrentIcon"=w578, "RenameOption.BgColor"=w546, "RenameOption.IconOut"=w545, "RowStart(0)"=w549, "ImageRows(32)"=w548) -> (w561:T6)
        n269 = local write "_After"(w560) -> ()
        n270 = local write "_IconPreview"(w559) -> ()
      }
      frame "", "Idle" {
        n271 = event shown="[0] \"NewName\": Value Change" {
          selector: _ -> [_ _ _ _ _ _ _ _ _ _ _ _ _ _ _]
          dyn-events: _ -> [_ _ _ _ _ _ _ _ _ _ _ _ _ _ _]
          timeout: _ -> [_ _ _ _ _ _ _ _ _ _ _ _ _ _ _]
          tunnel: w582 -> [w593 w609 w657 w674 w687 w700 w756 w761 w794 w800 w828 w833 w836 w838 w843]
          tunnel: [w592 w608 w658 w672 w685 w699 w756 w760 w793 w799 w828 w832 w836 w838 w841] -> w584
          tunnel: ["UpdateSelection\nGenerateIcon" w607 w653 "Exit" "GenerateIcon\nExit" w701 "GenerateIcon" w759 _ w803 _ "Exit" _ _ _] -> w583
          tunnel: w582 -> [w587 w606 _ _ w679 w698 _ w758 w795 w802 w827 _ _ _ _]
          tunnel: w581 -> [w585 w611 w652 w670 w682 w696 w754 w757 w792 w798 w823 w830 w835 w837 w842]
          tunnel: [w585 w610 w652 w670 w682 w696 w754 w757 w792 w798 w823 w830 w835 w837 w842] -> w580
          event "NewName": Value Change {
            n272 = event-data() -> ()  [unwired: 1 in, 1 out]
            n273 = Unbundle By Name(w587) -> ("FileExtension"=w586:string)
            n274 = call <vilib>:"Trim Whitespace.vi"("string"="NewName") -> ("trimmed string"=w589:string)  [unwired: 1 in]
            n275 = Empty String/Path?(string/path=w589) -> (empty?=w588:bool)
            n276 = case shown="False" w588 {
              tunnel: [w599 _] -> w590
              tunnel: w589 -> [w595 _]
              tunnel: w586 -> [w597 _]
              frame False {
                n277 = Match Pattern(string=w595, regular expression="\\2E[A-Za-z]+$") -> (before substring=w598:string, offset past match=w596:i32)  [unwired: 1 in, 2 out]
                n278 = local write "_MethodIconName"(w598) -> ()
                n279 = case shown="0, Default" w596 {
                  tunnel: [w601 w604] -> w599
                  tunnel: w598 -> [_ w603]
                  tunnel: w597 -> [_ w602]
                  tunnel: w595 -> [w601 _]
                  frame 0, Default {
                  }
                  frame -1 {
                    n280 = Concatenate Strings(w603, "." ("string"), w602) -> (w604:string)
                  }
                }
              }
              frame True {
              }
            }
            n281 = Bundle By Name(cluster=w593, "NewName"=w590) -> (w592:T6)
          }
          event "_MethodIcons": Value Change {
            n282 = event-data() -> ()  [unwired: 1 in, 1 out]
            n283 = Unbundle By Name(w606) -> ("HeaderIcon"=w636:u8[][])
            n284 = Unbundle By Name(w606) -> ("RowStart(0)"=w632:i32, "ImageRows(32)"=w631:i32, "Frame thickness"=w633:i32, "FrameColor"=w630:u32)
            n285 = Unbundle By Name(w606) -> ("BodyIconHeight"=w621:i32, "BodyIconWidth"=w620:i32, "HeaderBkColor"=w619:u32, "Offset"=w613:cluster{"X":i32, "Y":i32}, "CurrentIcon"=w612:T17)
            n286 = local read "_IconSize"() -> (w641:u16)
            n287 = local read "_HideHeader"() -> (w638:bool)
            n288 = local read "_BodyBk"() -> (w625:T2)
            n289 = local read "_BodyText"() -> (w624:T2)
            n290 = Equal?(x=w641, y=u16 1) -> (x = y?=w639:bool)
            n291 = local read "_MethodIconName"() -> (w629:string)
            n292 = local read "_FontCompression"() -> (w627:enum16{"Auto", "On", "Off"})
            n293 = local read "_TextAlignment"() -> (w626:u16)
            n294 = local read "_CapitalOnly"() -> (w628:bool)
            n295 = Or(x=w638, y=w639) -> (x .or. y?=w637:bool)
            n296 = Unbundle By Name(w624) -> ("Color"=w623:u32)
            n297 = Unbundle By Name(w625) -> ("Color"=w622:u32)
            n298 = Select(t=u8[][] [], s=w637, f=w636) -> (s? t:f=w634:u8[][])
            n299 = Bundle By Name(cluster=T14 {"HeaderIcon"=[], "RowStart(0)"=0, "ImageRows(32)"=32, "FrameThickness(1)"=1, "FrameColor"=0, "IconTextDataType"={"Text"="", "Allow Only Capital Chars"=FALSE, "Compression"=enum."Auto", "Alignment"=enum."Center"}, "BodyTextColor"=0, "BodyBackgroundColor"=0, "BodyIconHeight"=0, "BodyIconWidth"=0, "HeaderBackgroundColor"=0, "BodyIcon"=[[0, 0, 0, 0, 0, 0, 0, 0, 0, 0, 255, 255, 0, 0, 255, 0, 0, 0, 255, 0, 0, 0, 0, 0, 0, 0, 0, 0, 0, 0], [0, 0, 0, 0, 0, 0, 0, 0, 0, 255, 0, 0, 255, 0, 255, 0, 0, 0, 255, 0, 0, 0, 0, 0, 0, 0, 0, 0, 0, 0], [0, 0, 0, 0, 0, 0, 0, 0, 0, 255, 255, 255, 255, 0, 255, 0, 0, 0, 255, 0, 0, 0, 0, 0, 0, 0, 0, 0, 0, 0], [0, 0, 0, 0, 0, 0, 0, 0, 0, 255, 0, 0, 255, 0, 255, 0, 0, 0, 255, 0, 0, 0, 0, 0, 0, 0, 0, 0, 0, 0], [0, 0, 0, 0, 0, 0, 0, 0, 0, 255, 0, 0, 255, 0, 255, 255, 255, 0, 255, 255, 255, 0, 0, 0, 0, 0, 0, 0, 0, 0], [0, 0, 255, 0, 0, 0, 255, 0, 0, 255, 255, 0, 0, 255, 0, 0, 255, 0, 255, 255, 0, 255, 255, 0, 0, 0, 255, 255, 0, 0], [0, 255, 0, 255, 0, 255, 0, 255, 0, 255, 0, 255, 0, 255, 255, 0, 255, 0, 255, 0, 0, 255, 0, 255, 0, 255, 0, 0, 0, 0], [0, 255, 0, 0, 0, 255, 0, 255, 0, 255, 255, 0, 0, 255, 0, 255, 255, 0, 255, 255, 0, 255, 255, 0, 0, 0, 255, 0, 0, 0], [0, 255, 0, 255, 0, 255, 0, 255, 0, 255, 0, 255, 0, 255, 0, 0, 255, 0, 255, 0, 0, 255, 0, 255, 0, 0, 0, 255, 0, 0], [0, 0, 255, 0, 0, 0, 255, 0, 0, 255, 0, 255, 0, 255, 0, 0, 255, 0, 255, 255, 0, 255, 0, 255, 0, 255, 255, 0, 0, 0], [0, 255, 0, 0, 0, 255, 0, 0, 255, 0, 0, 255, 0, 255, 0, 0, 255, 0, 255, 255, 0, 0, 255, 0, 0, 255, 255, 255, 0, 255], [255, 0, 255, 0, 255, 0, 255, 0, 255, 255, 0, 255, 0, 255, 255, 0, 255, 0, 255, 0, 0, 255, 0, 255, 0, 0, 255, 0, 0, 255], [255, 0, 0, 0, 255, 0, 255, 0, 255, 0, 255, 255, 0, 255, 0, 255, 255, 0, 255, 255, 0, 255, 0, 0, 0, 0, 255, 0, 0, 255], [255, 0, 255, 0, 255, 0, 255, 0, 255, 0, 0, 255, 0, 255, 0, 0, 255, 0, 255, 0, 0, 255, 0, 255, 0, 0, 255, 0, 0, 255], [0, 255, 0, 0, 0, 255, 0, 0, 255, 0, 0, 255, 0, 255, 0, 0, 255, 0, 255, 255, 0, 0, 255, 0, 0, 0, 255, 0, 0, 255], [0, 0, 0, 0, 0, 0, 0, 0, 0, 0, 0, 0, 0, 0, 255, 0, 0, 0, 0, 0, 0, 0, 0, 0, 0, 0, 0, 0, 0, 0], [0, 0, 0, 0, 0, 0, 0, 0, 0, 0, 0, 0, 0, 255, 0, 0, 0, 0, 0, 0, 0, 0, 0, 0, 0, 0, 0, 0, 0, 0], [0, 0, 0, 0, 0, 0, 0, 0, 0, 0, 0, 0, 0, 255, 255, 0, 0, 0, 0, 0, 0, 0, 0, 0, 0, 0, 0, 0, 0, 0], [0, 0, 0, 0, 0, 0, 0, 0, 0, 0, 0, 0, 0, 255, 0, 255, 0, 0, 0, 0, 0, 0, 0, 0, 0, 0, 0, 0, 0, 0], [0, 0, 0, 0, 0, 0, 0, 0, 0, 0, 0, 0, 0, 0, 255, 0, 0, 0, 0, 0, 0, 0, 0, 0, 0, 0, 0, 0, 0, 0], [0, 0, 0, 0, 0, 0, 0, 0, 0, 0, 0, 0, 0, 0, 0, 0, 0, 0, 0, 0, 0, 0, 0, 0, 0, 0, 0, 0, 0, 0], [0, 0, 0, 0, 0, 0, 0, 0, 0, 0, 0, 0, 0, 0, 0, 0, 0, 0, 0, 0, 0, 0, 0, 0, 0, 0, 0, 0, 0, 0]], "Offset"={"X"=0, "Y"=0}, "CurrentIcon"={"BgIcon"=[], "BgIconOffset"={"X"=0, "Y"=0}, "BgIconMask"=[], "ColorsOkayforiconToBeOnTopOf"=[]}} ("IconInfo"), "HeaderIcon"=w634, "RowStart(0)"=w632, "ImageRows(32)"=w631, "FrameThickness(1)"=w633, "FrameColor"=w630, "IconTextDataType.Text"=w629, "IconTextDataType.Allow Only Capital Chars"=w628, "IconTextDataType.Compression"=w627, "IconTextDataType.Alignment"=w626, "BodyTextColor"=w623, "BodyBackgroundColor"=w622, "BodyIconHeight"=w621, "BodyIconWidth"=w620, "HeaderBackgroundColor"=w619, "Offset"=w613, "CurrentIcon"=w612) -> (w642:T14)
            n300 = call <resource>:"GDSIconEditor_IconDialog.vi"("error in (no error)"=w611, "IconInfo"=w642) -> ("error out"=w610:errorcluster, "Icon exist"=w614:bool, "CurrentIcon"=w615:T17, "Cancelled"=w616:bool, "Offset"=w617:cluster{"X":i32, "Y":i32}, "BodyIcon"=w618:u8[][])  [unwired: 4 in]
            n301 = case shown="False" w616 {
              tunnel: w609 -> [w650 w651]
              tunnel: [w649 w651] -> w608
              tunnel: w618 -> [w648 _]
              tunnel: w617 -> [w647 _]
              tunnel: w615 -> [w646 _]
              tunnel: w614 -> [w645 _]
              tunnel: ["GenerateIcon" _] -> w607
              frame False {
                n302 = Bundle By Name(cluster=w650, "BodyIcon"=w648, "Offset"=w647, "CurrentIcon"=w646, "Icon exist"=w645) -> (w649:T6)
              }
              frame True {
              }
            }
          }
          event "VIs to rename": Mouse Down {
            n303 = event-data() -> ("Coords"=w659:T4)  [unwired: 1 in, 7 out]
            n304 = invoke on="VIs to rename" class="MCListbox (strict)" method="Point To Row Column"("Point"=w659) -> ("CellPosition"=w656:T8, "InGlyph"=w654:bool)  [unwired: 6 in, 5 out]
            n305 = Unbundle By Name(w656) -> ("Row"=w655:i32)
            n306 = case shown="True" w654 {
              tunnel: [w660 w664] -> w658
              tunnel: w657 -> [w660 w663]
              tunnel: w655 -> [_ w662]
              tunnel: [_ "UpdateSelection"] -> w653
              frame False {
              }
              frame True {
                n307 = in-place {
                  in-place-border: w662 -> [w665]
                  n308 = in-place-cluster #1(w663) -> ("SelectedItems"=w667:bool[])
                  n309 = in-place {
                    n310 = in-place-array #2(w667, w665) -> (w669:bool)
                    n311 = Not(x=w669) -> (.not. x?=w668:bool)
                    n312 = in-place-array #2(w668) -> (w666:bool[])  [unwired: 1 out]
                  }
                  n313 = in-place-cluster #1("SelectedItems"=w666) -> (w664:T6)
                }
              }
            }
          }
          event "_Cancel": Value Change {
            n314 = event-data() -> ()  [unwired: 1 in, 1 out]
            n315 = Bundle By Name(cluster=w674, "Cancelled"="_Cancel") -> (w672:T6)
          }
          event "_RenameVI": Value Change {
            n316 = event-data() -> ()  [unwired: 1 in, 1 out]
            n317 = Unbundle By Name(w679) -> ("VIPath"=w675:path, "ClassVIs"=w680:T15, "InterfaceVIs"=w681:T15, "SelectedItems"=w677:bool[])
            n318 = Unbundle By Name(w679) -> ("NewName"=w684:string)
            n319 = Build Array (concatenate)(w680, w681) -> (w678:T15)
            n320 = Empty Array?(array=w677) -> (empty?=w676:bool)
            n321 = case shown="True" w676 {
              tunnel: [w690 w694] -> w683
              tunnel: w678 -> [w689 _]
              tunnel: w677 -> [w688 _]
              tunnel: w675 -> [_ w695]
              frame False {
                n322 = for {
                  tunnel: w689 -> [w692] mode=indexing
                  tunnel: [w693] -> w690 mode=indexing if=w691
                  tunnel: w688 -> [w691] mode=indexing
                  n323 = Unbundle By Name(w692) -> ("ViFullPath"=w693:path)
                }
              }
              frame True {
                n324 = Build Array(w695) -> (w694:path[])
              }
            }
            n325 = Bundle By Name(cluster=w687, "RenameOption.NewVIName"=w684, "RenameOption.VIs"=w683) -> (w685:T6)
          }
          event Key Down? {
            (unwired) TRUE
            n326 = event-data() -> ("VKey"=w704:T19, "PlatMods"=w703:T20)  [unwired: 1 in, 3 out]
            n327 = property on="_FontCompression" class="Enum (strict)"() -> ("Key Focus"=w707:bool)  [unwired: 2 in, 2 out]
            n328 = property on="_MethodIconName" class="Str"() -> ("Key Focus"=w710:bool)  [unwired: 2 in, 2 out]
            n329 = property on="NewName" class="Str"() -> ("Key Focus"=w697:bool)  [unwired: 2 in, 2 out]
            n330 = property on="_TextAlignment" class="Ring (strict)"() -> ("Key Focus"=w709:bool)  [unwired: 2 in, 2 out]
            n331 = property on="_IconSize" class="Ring (strict)"() -> ("Key Focus"=w708:bool)  [unwired: 2 in, 2 out]
            n332 = Compound Arithmetic op=AND(invert w707, invert w708, invert w709, invert w710, invert w697) -> (w711:bool)
            n333 = Unbundle By Name(w698) -> ("Offset.X"=w706:i32, "Offset.Y"=w705:i32)
            n334 = Unbundle By Name(w703) -> ("Ctrl"=w712:bool)
            n335 = Or(x=w712, y=w711) -> (x .or. y?=w713:bool)
            n336 = case shown="True" w713 {
              tunnel: w700 -> [w715 w719]
              tunnel: [w715 w723] -> w699
              tunnel: w704 -> [_ w722]
              tunnel: w705 -> [_ w716]
              tunnel: w706 -> [_ w717]
              tunnel: ["Idle" w721] -> w701
              tunnel: [_ w720] -> w702
              frame False {
              }
              frame True {
                n337 = Bundle By Name(cluster=w719, "OldOffset.X"=w717, "OldOffset.Y"=w716) -> (w718:T6)
                n338 = case shown="\"Right\"" w722 {
                  tunnel: w718 -> [w730 w732 w734 w741 w748]
                  tunnel: [w729 w732 w733 w740 w747] -> w723
                  tunnel: w716 -> [w728 _ w739 w742 w749]
                  tunnel: w717 -> [w726 _ w735 w746 w753]
                  tunnel: ["GenerateIcon" "Idle" "GenerateIcon" "GenerateIcon" "GenerateIcon"] -> w721
                  tunnel: [TRUE _ TRUE TRUE TRUE] -> w720
                  frame "Up" {
                    n339 = Decrement(x=w728) -> (x-1=w727:i32)
                    n340 = Bundle By Name(cluster=w730, "Offset.X"=w726, "Offset.Y"=w727) -> (w729:T6)
                  }
                  frame Default {
                  }
                  frame "Down" {
                    n341 = Increment(x=w739) -> (x+1=w736:i32)
                    n342 = Bundle By Name(cluster=w734, "Offset.X"=w735, "Offset.Y"=w736) -> (w733:T6)
                  }
                  frame "Left" {
                    n343 = Decrement(x=w746) -> (x-1=w743:i32)
                    n344 = Bundle By Name(cluster=w741, "Offset.X"=w743, "Offset.Y"=w742) -> (w740:T6)
                  }
                  frame "Right" {
                    n345 = Increment(x=w753) -> (x+1=w750:i32)
                    n346 = Bundle By Name(cluster=w748, "Offset.X"=w750, "Offset.Y"=w749) -> (w747:T6)
                  }
                }
              }
            }
            n347 = event-data("Discard?"=w702) -> ()  [unwired: 1 in, 1 out]
          }
          event "_MethodIconName", "_TextAlignment", "_FontCompression", "_HideHeader", "_IconSize", "_CapitalOnly": Value Change {
            n348 = event-data() -> ()  [unwired: 1 in, 1 out]
          }
          event "_IconPreview": Mouse Down {
            w775 = 4 ("y")
            n349 = event-data() -> ("Coords"=w762:T4)  [unwired: 1 in]
            n350 = property on="_IconPreview" class="Pict"() -> ("Mouse"=w771:T21)  [unwired: 2 in, 2 out]
            n351 = Unbundle By Name(w771) -> ("Mouse Position.X"=w774:i32, "Mouse Position.Y"=w772:i32)
            n352 = Unbundle By Name(w758) -> ("IconDropped"=w763:i32, "TextBounds"=w764:T18)
            n353 = Unbundle(w764) -> ("FirstRow"=w766:i32, "FirstColumn"=w767:i32, "LastRow"=w765:i32, "LastColumn"=w770:i32)
            n354 = Divide(x=w774, y=w775) -> (x/y=w776:dbl)
            n355 = Divide(x=w772, y=w775) -> (x/y=w773:dbl)
            n356 = In Range and Coerce(upper limit=w765, x=w773, lower limit=w766) -> (In Range?=w768:bool)  [unwired: 1 out]
            n357 = In Range and Coerce(upper limit=w770, x=w776, lower limit=w767) -> (In Range?=w769:bool)  [unwired: 1 out]
            n358 = And(x=w768, y=w769) -> (x .and. y?=w777:bool)
            n359 = case shown="True" w777 {
              tunnel: w761 -> [w779 w791]
              tunnel: [w779 w789] -> w760
              tunnel: ["Idle" ("y") "Idle" ("y")] -> w759
              tunnel: w762 -> [_ w783]
              tunnel: w763 -> [_ _]
              tunnel: w758 -> [_ w787]
              frame False {
              }
              frame True {
                n360 = Unbundle By Name(w787) -> ("Offset.X"=w786:i32, "Offset.Y"=w785:i32)
                n361 = Bundle("X"=w786, "Y"=w785) -> (w781:cluster{"X":i32, "Y":i32})  [unwired: 1 in]
                n362 = Multiply(x=w781, y=4) -> (x*y=w780:cluster{"X":i32, "Y":i32})
                n363 = Subtract(x=w783, y=w780) -> (x-y=w782:T4)
                n364 = Bundle By Name(cluster=w791, "DraggingText"=TRUE, "StartTextDraggingPos"=w782) -> (w789:T6)
              }
            }
          }
          event "_IconPreview": Mouse Up {
            n365 = event-data() -> ()  [unwired: 1 in, 3 out]
            n366 = Unbundle By Name(w795) -> ("IconSelected"=w797:i32)
            n367 = Bundle By Name(cluster=w794, "IconDropped"=w797, "Moving"=FALSE ("Draging")) -> (w793:T6)
          }
          event Mouse Move {
            n368 = event-data() -> ("Coords"=w801:T4)  [unwired: 1 in]
            n369 = Unbundle By Name(w802) -> ("StartTextDraggingPos"=w805:T4)
            n370 = Unbundle By Name(w802) -> ("DraggingText"=w804:bool)
            n371 = case shown="True" w804 {
              tunnel: w800 -> [w807 w822]
              tunnel: [w807 w821] -> w799
              tunnel: [_ "GenerateIcon"] -> w803
              tunnel: w805 -> [_ w818]
              tunnel: w801 -> [_ w819]
              tunnel: w802 -> [_ w817]
              frame False {
                n372 = property on="NewName" class="Str"() -> ("Key Focus"=w806:bool)  [unwired: 2 in, 2 out]
                n373 = case shown="False" w806 {
                  selector: w806 -> [w808 _]
                  frame False {
                    n374 = property on="Ballon" class="Clust (strict)"("Visible"=w808) -> ()  [unwired: 2 in, 2 out]
                  }
                  frame True {
                  }
                }
              }
              frame True {
                n375 = Subtract(x=w819, y=w818) -> (x-y=w814:T4)
                n376 = Unbundle By Name(w817) -> ("Offset.X"=w812:i32, "Offset.Y"=w811:i32)
                n377 = Divide(x=w814, y=u8 4 ("f")) -> (x/y=w813:cluster{"Horizontal":dbl, "Vertical":dbl})
                n378 = Unbundle By Name(w813) -> ("Horizontal"=w810:dbl, "Vertical"=w809:dbl)
                n379 = Bundle By Name(cluster=w822, "OldOffset.X"=w812, "OldOffset.Y"=w811) -> (w816:T6)
                n380 = Bundle By Name(cluster=w816, "Offset.X"=w810, "Offset.Y"=w809) -> (w821:T6)
              }
            }
          }
          event "Ballon": Mouse Enter {
            n381 = event-data() -> ()  [unwired: 1 in, 4 out]
            n382 = Unbundle By Name(w827) -> ("StartTime"=w826:i32)
            n383 = Tick Count (ms)() -> (millisecond timer value=w825:u32)
            n384 = Subtract(x=w825, y=w826) -> (x-y=w824:u32)
            n385 = case shown="3000.." w824 {
              frame 0, Default {
              }
              frame 3000.. {
                n386 = property on="Ballon" class="Clust (strict)"("Visible"=FALSE) -> ()  [unwired: 2 in, 2 out]
              }
            }
          }
          event Panel Close? {
            w831 = TRUE ("Discard?")
            n387 = event-data() -> ()  [unwired: 1 in, 1 out]
            n388 = Bundle By Name(cluster=w833, "Cancelled"=w831) -> (w832:T6)
            n389 = event-data("Discard?"=w831) -> ()  [unwired: 1 in, 1 out]
          }
          event "Help": Value Change {
            n390 = event-data() -> ()  [unwired: 1 in, 6 out]
            n391 = call <resource>:"GOOP_HelpMain.vi"() -> ()  [unwired: 12 in]
          }
          event "_ShowContextHelp": Value Change {
            n392 = event-data() -> ("NewVal"=w839:bool)  [unwired: 1 in]
            n393 = Control Help Window(1:w839) -> ()  [unwired: 1 in]
          }
          event Mouse Up; Mouse Leave {
            n394 = event-data() -> ()  [unwired: 1 in, 4 out]
            n395 = Bundle By Name(cluster=w843, "DraggingText"=FALSE) -> (w841:T6)
          }
        }
      }
    }
  }
  "error out" <- w15
  n396 = Unbundle By Name(w17) -> ("Cancelled"=→"Cancelled":bool, "RenameOption"=→"RenameOption":T1)
  n397 = call <resource>:"GDSString_AddStatesToQueue.vi"() -> ()  [unwired: 15 in, 1 out]
  "ObjectOut" <- "ObjectIn"
